vi "01_ui_main_loop.vi"() -> ()   [LabVIEW 2025]
uses:
  0417e9bc-26c0-40a3-857c-749a2451377f.vi
  040e489e-a473-4f93-bd06-0afa5652ce70.vi
  c6e3c1e2-0994-45fa-bff3-5cd5cb70e039.vi
  0bc7f4c2-ffb1-4822-9f64-357063f019c3.vi
  8b609e5e-a51d-4c52-8c18-d6a58a5b9e80.vi
  43d63275-3364-44ab-a9c8-6f7e055a0a8e.vi
  75836779-3642-44ab-91a1-288c14d5bff7.vi
  f856a27e-8979-4d67-ac65-7e3e0066168f.vi
  f6c46c24-e81c-4bed-970f-882e3bbfa33a.vi
  674b8dbc-10ac-464c-a410-8119d69976f5.vi
  efe7b7fb-95db-4648-be1d-36dd24965d64.vi
  a7921508-b016-4ad4-9c73-64ec30acdca8.vi
  2bf2835e-c011-4d5e-a055-403be64c671f.vi
  <vilib>/Utility/config.llb/Read Key (String).vi
  <vilib>/Utility/config.llb/Read Key (U32).vi
  <vilib>/Utility/config.llb/Read Key (Boolean).vi
  <vilib>/Utility/config.llb/Write Key (String).vi
  <vilib>/Utility/config.llb/Write Key (U32).vi
  <vilib>/Utility/config.llb/Write Key (Boolean).vi
  <vilib>/Utility/config.llb/NI_LVConfig.lvlib
panel:
  in  "color_picker_cursor_2":u32(colorbox)=16756736
  in  "color_picker_cursor_1":u32(colorbox)=11927752
  in  "sva_del_cal_file":bool
  in  "sva_cal_file":string(combo)
  in  "button_tcp_load_cal":bool caption="Connect"
  in  "button_tcp_smith_mode":bool caption="Connect"
  in  "button_tcp_s21_mode":bool caption="Connect"
  in  "button_tcp_s11_mode":bool caption="Connect"
  in  "button_tcp_vna_mode":bool caption="Connect"
  in  "show_plot_window":bool
  in  "button_save_s2p":bool caption="Save *.s2p"
  in  "button_tcp_connect":bool caption="Connect"
  in  "sva_port":u16=5025 caption="Port"
  in  "sva_ip":string="192.168.2.29" caption="IP"
  in  "stop":bool
  in  "button_auto_sweep":bool caption="Auto Sweep"
  in  "sweep_points":dbl caption="Points" min=0.0 step=1.0 format="%#_6f"
  in  "sweep_stop":dbl caption="Stop Frequency" min=0.0 step=1.0 format="%#_6f"
  in  "sweep_start":dbl caption="Start Frequency" min=0.0 step=1.0 format="%#_6f"
  in  "selector_serial_port":refnum<visa-resource-name>="COM1" caption="COM-Port"
  out "led_serial_connected":bool caption="Connected"
  in  "button_serial_connect":bool caption="Connect"
  in  "button_single_sweep":bool caption="Single Sweep"
  out "plot_smith_legend_curs_r":dbl caption="Cursor - R"
  out "plot_smith_legend_phase":dbl caption="Phase"
  out "plot_smith_legend_freq":string caption="Frequency"
  out "plot_smith_legend_jx":dbl caption="jX"
  out "plot_smith_legend_r":dbl caption="R"
  out "plot_smith":picture caption="Smith"
  out "filename":string caption="Recent File"
  in  "button_save_s1p":bool caption="Save *.s1p"
  in  "button_load_csv":bool caption="Load *.s1p 2"
  in  "button_load_sxp":bool caption="Load *.sxp"
  in  "show_smith_window":bool
  out "min_vswr_idx":i32
  in  "set_min_vswr_c2":bool
  in  "set_min_vswr_c1":bool
  out "min_vswr_freq":string caption="@ Frequency"
  out "min_vswr":dbl caption="Min. VSWR"
  out "min_frequency":string caption="Min. Frequency"
  out "points":dbl caption="Points"
  out "max_frequency":string caption="Max. Frequency"
  out "plot_smith_legend_curs_x":dbl caption="Cursor - jX"
  out "cursor_cp_1_prefix":string
  out "cursor_lp_1_prefix":string
  out "cursor_cs_1_prefix":string
  out "cursor_ls_1_prefix":string
  out "cursor_cp_2_prefix":string
  out "cursor_lp_2_prefix":string
  out "cursor_cs_2_prefix":string
  in  "lc_scale_settings":enum32{"autoscale", "fancy_scale", "zero_scale"}(radio)=enum."zero_scale"
  out "cursor_ls_2_prefix":string
  out "cursor_cp_2":dbl format="%#_6f"
  in  "color_picker_cp":u32(colorbox)=14468608
  out "cursor_cp_1":dbl format="%#_6f"
  in  "enable_plot_cp":bool=TRUE caption="S11 - Imaginary"
  out "cursor_lp_2":dbl format="%#_6f"
  in  "color_picker_lp":u32(colorbox)=39219
  out "cursor_lp_1":dbl format="%#_6f"
  in  "enable_plot_lp":bool caption="S11 - Imaginary"
  out "cursor_cs_2":dbl format="%#_6f"
  out "cursor_ls_2":dbl format="%#_6f"
  out "cursor_lc_freq_2":string caption="Frequenz"
  out "cursor_lc_wavel_2":dbl caption="Frequenz"
  out "cursor_lc_wavel_1":dbl caption="Frequenz"
  in  "color_picker_cs":u32(colorbox)=14423100
  in  "color_picker_ls":u32(colorbox)=26316
  out "cursor_lc_freq_1":string caption="Frequenz"
  out "cursor_cs_1":dbl format="%#_6f"
  out "cursor_ls_1":dbl format="%#_6f"
  in  "enable_plot_cs":bool caption="S11 - Imaginary"
  in  "enable_plot_ls":bool=TRUE caption="S11 - Real"
  out "plot_lc":cluster{"array type (2D Dbl)":dbl[], dbl[]}[](graph) caption="L+C (Serial) / Lp+Cp (Parallel)"
  out "cursor_z_2":dbl format="%#_6f"
  in  "color_picker_z":u32(colorbox)=13314815
  out "cursor_z_1":dbl format="%#_6f"
  in  "enable_plot_z":bool=TRUE caption="S11 - Imaginary"
  out "cursor_jxp_2":dbl format="%#_6f"
  in  "color_picker_jxp":u32(colorbox)=14468608
  out "cursor_jxp_1":dbl format="%#_6f"
  in  "enable_plot_jxp":bool caption="S11 - Imaginary"
  out "cursor_rp_2":dbl format="%#_6f"
  in  "color_picker_rp":u32(colorbox)=39219
  out "cursor_rp_1":dbl format="%#_6f"
  in  "enable_plot_rp":bool caption="S11 - Imaginary"
  out "cursor_jx_2":dbl format="%#_6f"
  out "cursor_r_2":dbl format="%#_6f"
  out "cursor_imag_2":dbl format="%#_6f"
  out "cursor_real_2":dbl format="%#_6f"
  out "cursor_r_jx_freq_2":string caption="Frequenz"
  out "cursor_r_jx_wavel_2":dbl caption="Frequenz"
  out "cursor_r_jx_wavel_1":dbl caption="Frequenz"
  out "cursor_real_imag_freq_2":string caption="Frequenz"
  out "cursor_real_imag_wavel_2":dbl caption="Frequenz"
  out "cursor_real_imag_wavel_1":dbl caption="Frequenz"
  out "cursor_log_phase_wavel_2":dbl caption="Frequenz"
  out "cursor_log_phase_wavel_1":dbl caption="Frequenz"
  in  "cursor_mode":bool=TRUE caption="Cursor Mode"
  out "cursor_vswr_2":dbl format="%#_6f"
  in  "color_picker_vswr":u32(colorbox)=39219
  out "cursor_vswr_1":dbl format="%#_6f"
  in  "enable_plot_vswr":bool=TRUE caption="S11 - VSWR"
  out "cursor_log_phase_freq_2":string caption="Frequenz"
  out "cursor_phase_2":dbl format="%#_6f"
  out "cursor_logmag_2":dbl format="%#_6f"
  in  "color_picker_jx":u32(colorbox)=14423100
  in  "color_picker_r":u32(colorbox)=26316
  out "cursor_r_jx_freq_1":string caption="Frequenz"
  out "cursor_jx_1":dbl format="%#_6f"
  out "cursor_r_1":dbl format="%#_6f"
  in  "enable_plot_jx":bool=TRUE caption="S11 - Imaginary"
  in  "enable_plot_r":bool=TRUE caption="S11 - Real"
  in  "color_picker_imag":u32(colorbox)=14423100
  in  "color_picker_real":u32(colorbox)=26316
  out "cursor_real_imag_freq_1":string caption="Frequenz"
  out "cursor_imag_1":dbl format="%#_6f"
  out "cursor_real_1":dbl format="%#_6f"
  in  "enable_plot_imag":bool=TRUE caption="S11 - Imaginary"
  in  "enable_plot_real":bool=TRUE caption="S11 - Real"
  out "plot_real_imag":cluster{"array type (2D Dbl)":dbl[], dbl[]}[](graph) caption="Real / Imaginary"
  in  "color_picker_phase":u32(colorbox)=14423100
  in  "color_picker_logmag":u32(colorbox)=26316
  out "cursor_log_phase_freq_1":string caption="Frequenz"
  out "cursor_phase_1":dbl format="%#_6f"
  out "cursor_logmag_1":dbl format="%#_6f"
  in  "rx_scale_settings":enum32{"autoscale", "fancy_scale"}(radio)=enum."fancy_scale"
  in  "enable_plot_phase":bool=TRUE caption="S11 - Phase"
  in  "enable_plot_logmag":bool=TRUE caption="S11 - Logmag"
  out "plot_rjx":cluster{"array type (2D Dbl)":dbl[], dbl[]}[](graph) caption="R+jX (Serial) / Rp+jXp (Parallel) / Z"
  out "plot_log_phase_vswr":cluster{"array type (2D Dbl)":dbl[], dbl[]}[](graph) caption="Logmag / Phase / VSWR"
  # "LabVNA - VNA/S-Parameter Software"
  # "by Robin Tönniges (DC7RT)"
  # "Hz"
  # "NanoVNA"
  # "Siglent SVA"
  # "Sweep"
  # "Trace Data"
  # "Load/Save"
  # "Cursor 1"
  # "Cursor 2"
  # "Frequency"
  # "Hz"
  # "Hz"
  # "Wavelength"
  # "m"
  # "m"
  # "Frequency"
  # "Hz"
  # "Hz"
  # "Wavelength"
  # "m"
  # "m"
  # "Hz"
  # "Frequency"
  # "Hz"
  # "Wavelength"
  # "m"
  # "m"
  # "Frequency [MHz]"
  # "Hz"
  # "Frequency"
  # "Hz"
  # "Wavelength"
  # "m"
  # "m"
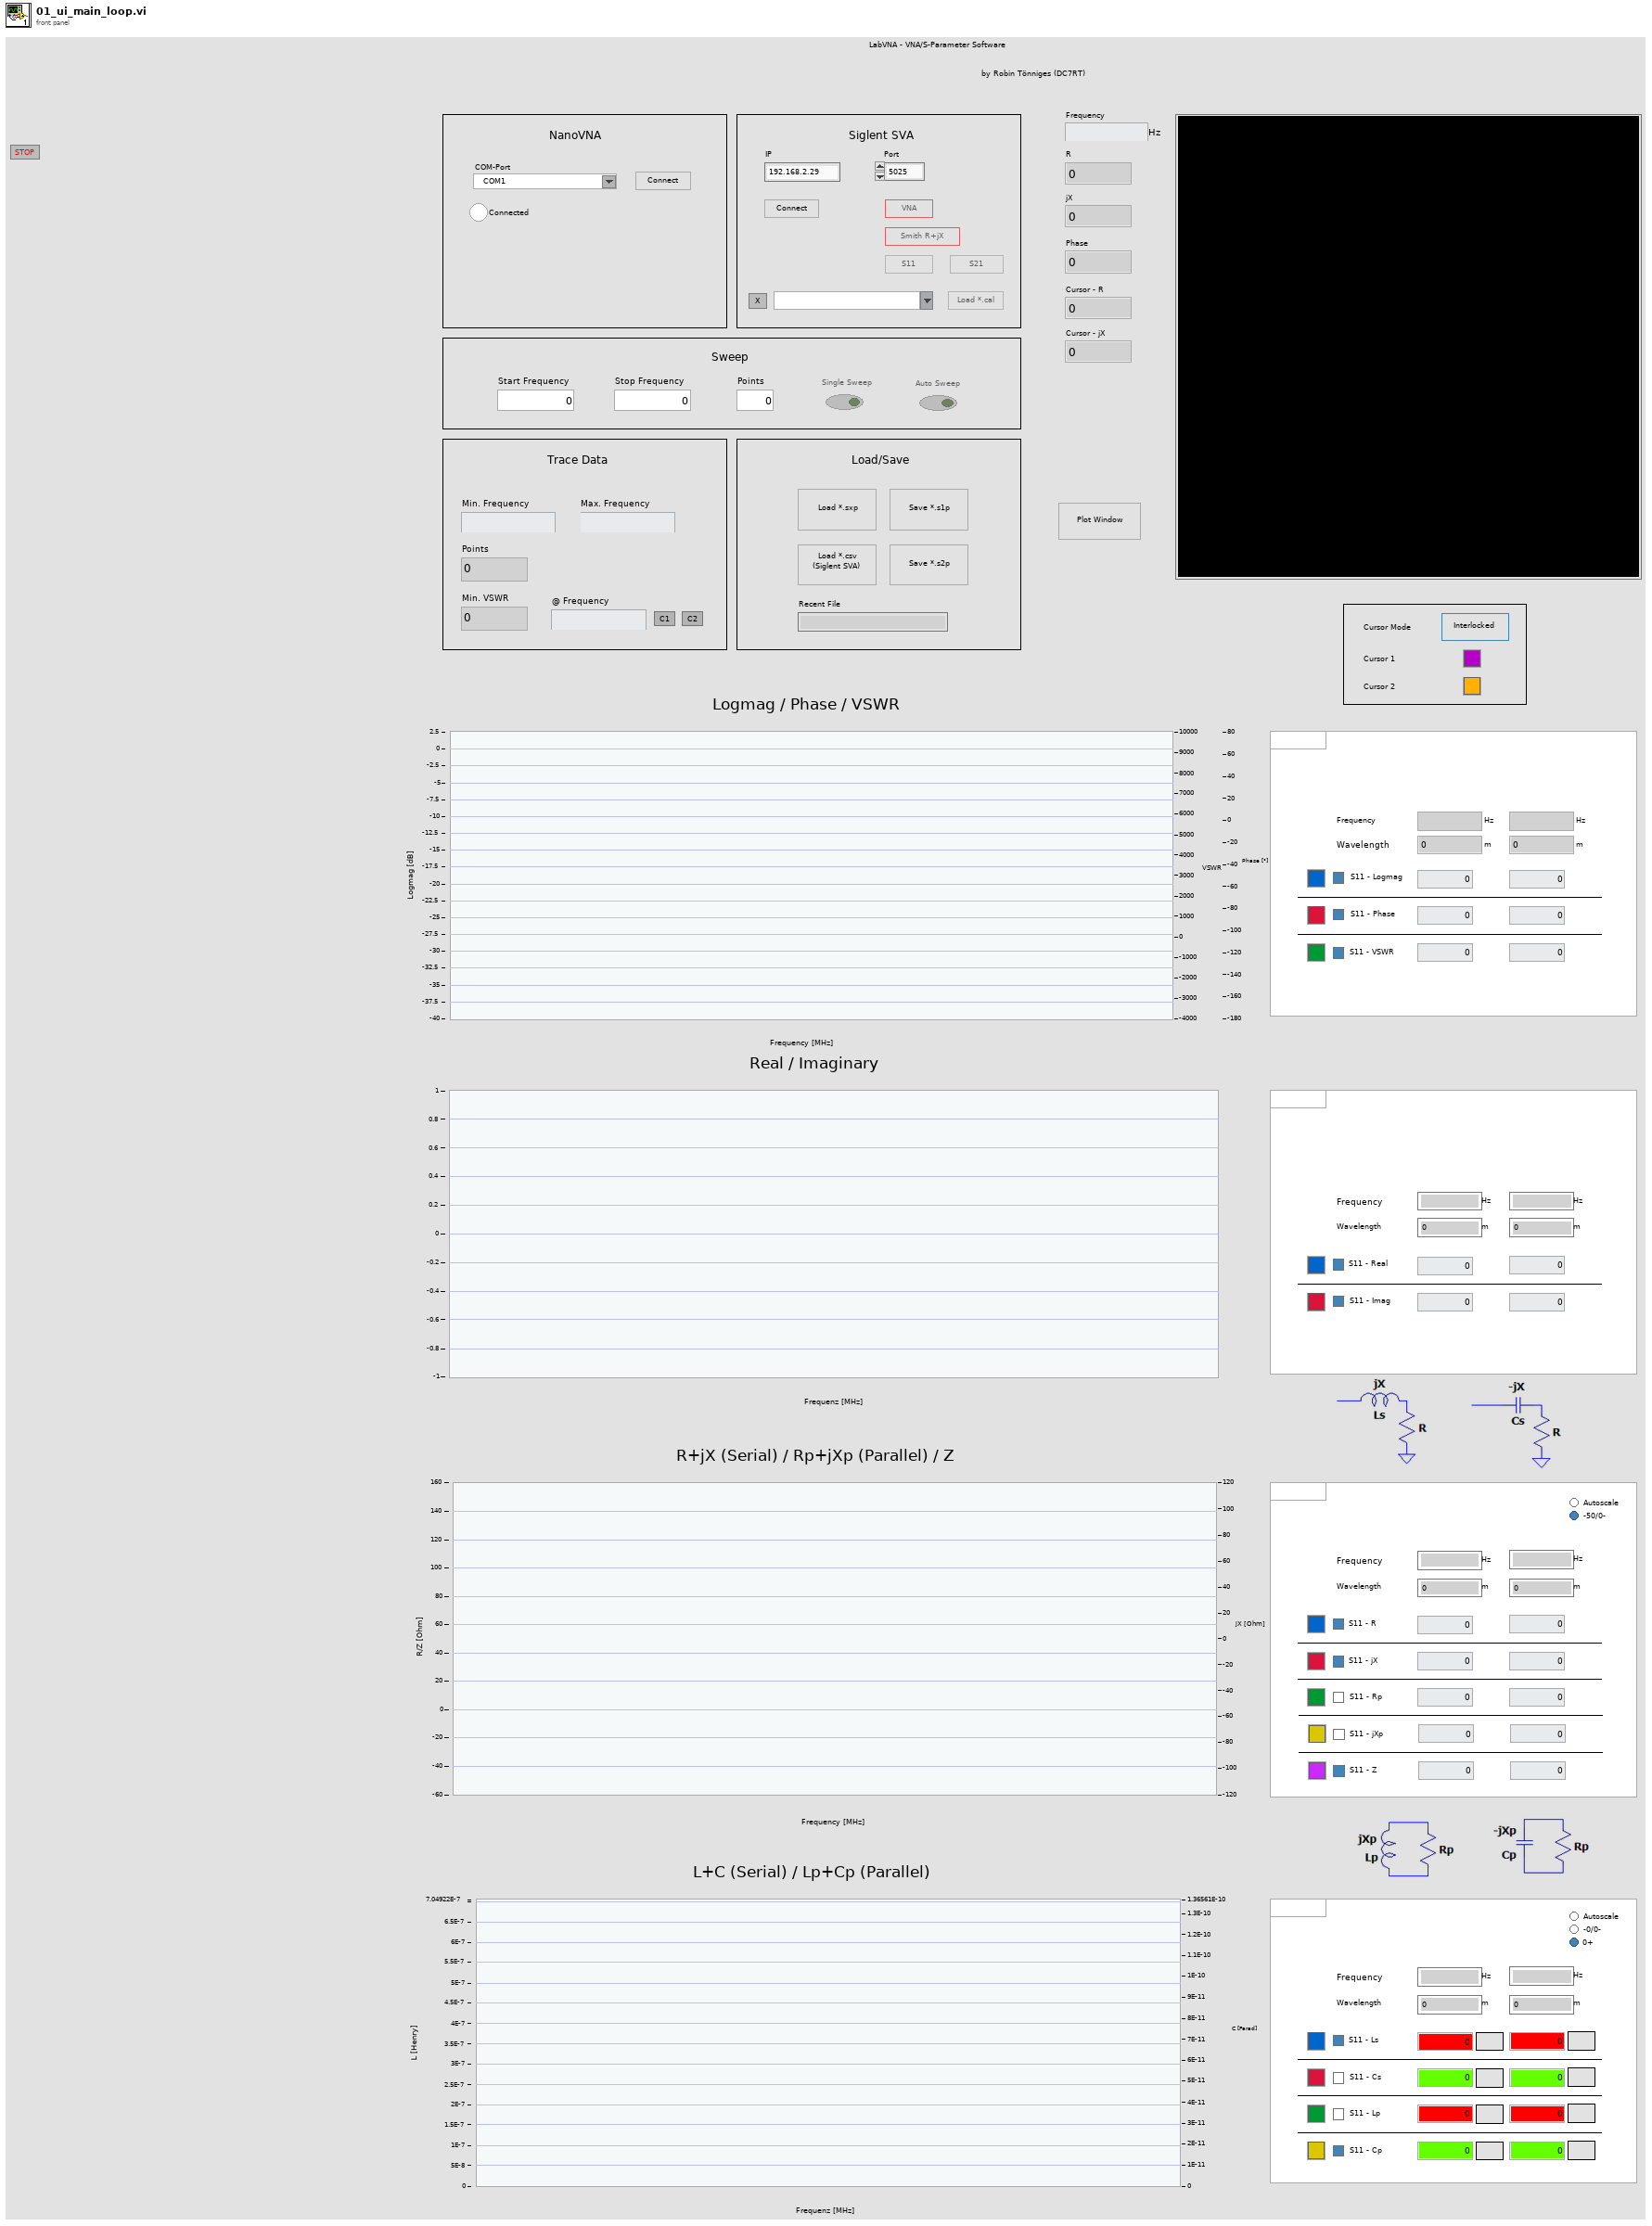
[diagram p1: front panel]
types:
  T1 = cluster{"button_serial_connect":bool, "button_auto_sweep":bool, "button_tcp_connect":bool}
  T2 = cluster{"button_load_sxp":bool, "button_load_csv":bool, "button_save_s1p":bool, "button_save_s2p":bool, "button_single_sweep":bool, "tcp_load_cal":bool, "show_smith_window":bool}
  T3 = enum8{"Enabled", "Disabled", "Disabled and Grayed Out"}
  T4 = enum32{"Invalid", "Standard", "Closed", "Hidden", "Minimized", "Maximized"}
  T5 = cluster{"left":dbl, "top":dbl, "right":dbl, "bottom":dbl}
  T6 = cluster{"x":cluster{"a":dbl, "b":dbl, "log?":bool}, "y":cluster{"a":dbl, "b":dbl, "log?":bool}}
  T7 = typedef "NI_LVConfig.lvlib/Config Data RefNum.ctl" = refnum<k1>
  T8 = cluster{"button_load_sxp":bool, "button_load_csv":bool, "button_save_s1p":bool, "button_save_s2p":bool, "button_single_sweep":bool, "button_tcp_load_cal":bool, "show_smith_window":bool}
  T9 = cluster{"mode":string, "s11_s21":string, "graph":string, "freq_range":cluster{"start_freq":string, "stop_freq":string}, "points":string}
  T10 = typedef "LVCursorListTypeDef.ctl" = cluster{"Name":string, "Color":u32, "Style":u8, "Point Style":u8, "Name Visible":bool, "Allow Drag":bool, "Cursor Mode":u32, "Plot":i32, "Index":i32, "Position":cluster{"X":dbl, "Y":dbl}, "X Scale":u32, "Y Scale":u32, "Watch Plots":i32[], "Watch All Plots":bool, "Plot Area":i32, "Label Offset":cluster{"X":dbl, "Y":dbl}}[]
  T11 = typedef "LVPoint32TypeDef.ctl" = cluster{"Horizontal":i32, "Vertical":i32}
  T12 = cluster{"frequency":dbl, "r":dbl, "jx":dbl, "phase":dbl}
  T13 = cluster{"cursor_data":dbl[], "frequency":string, "wavelength_m":dbl}
  T14 = cluster{"freq_array":dbl[], "data_array":dbl[]}[]
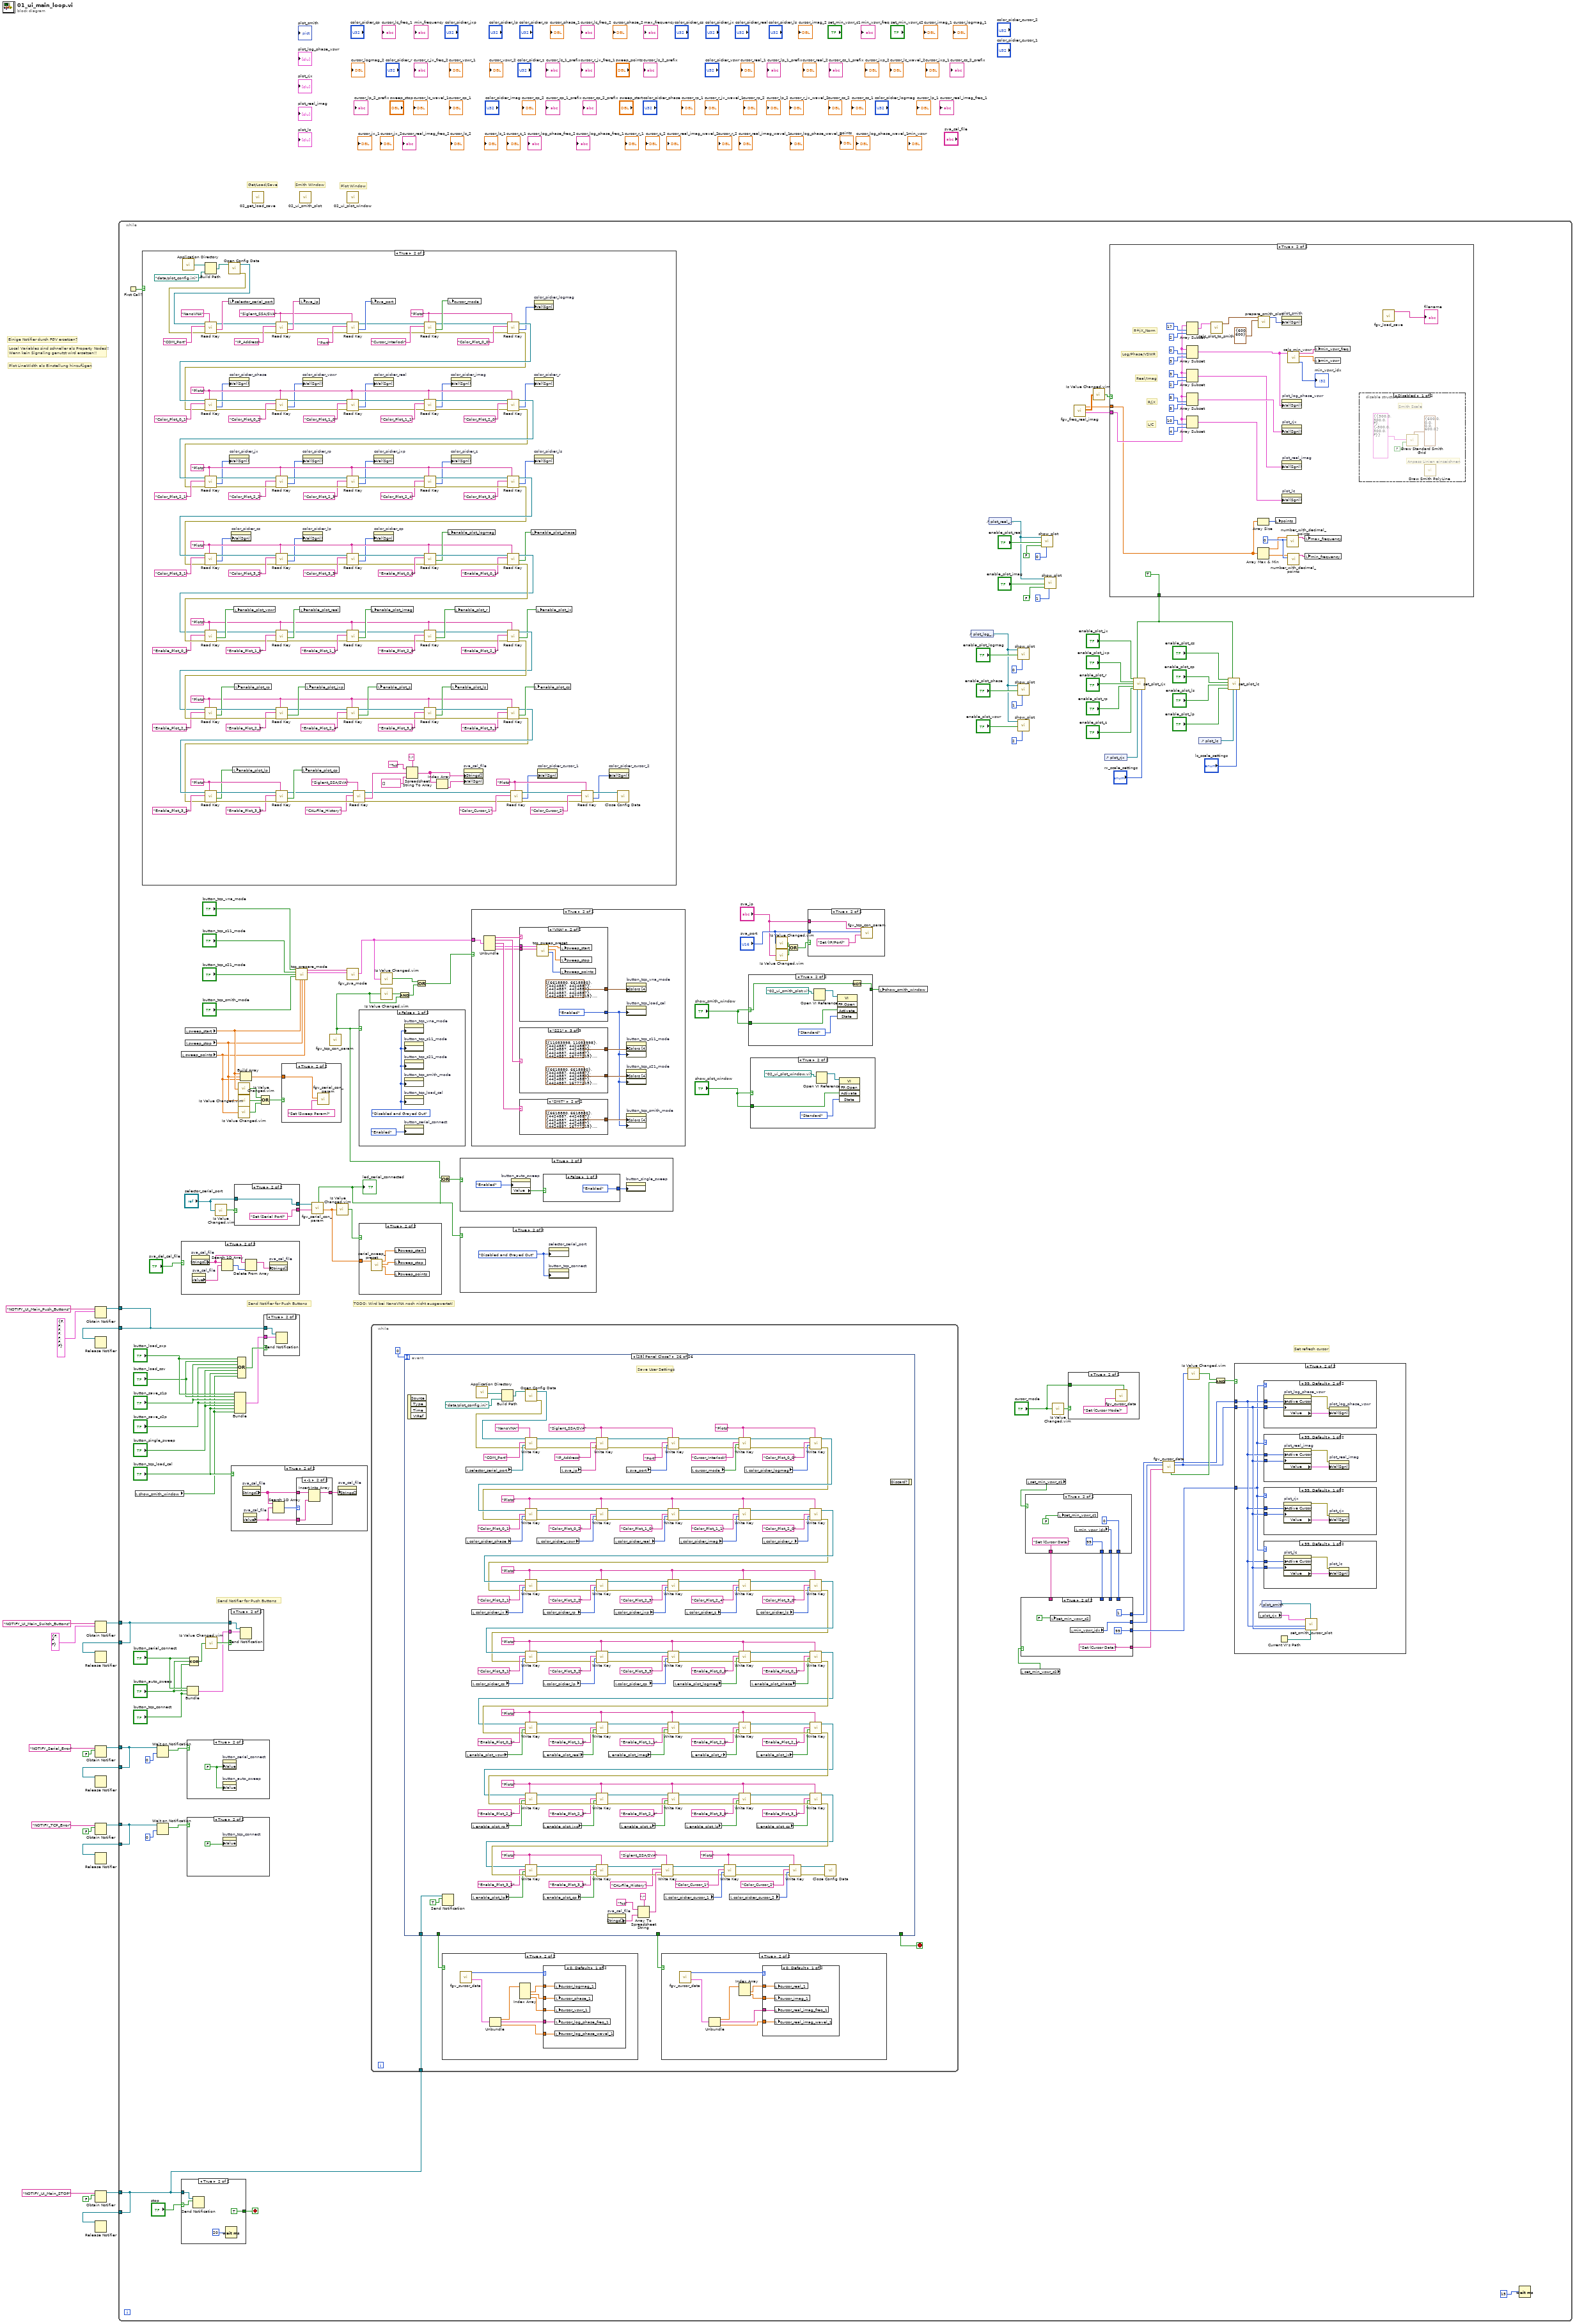
[diagram p0: block diagram]
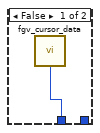
[diagram p9: hidden frame]
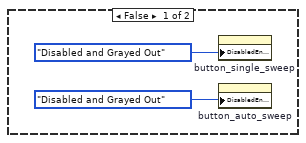
[diagram p11: hidden frame]
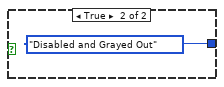
[diagram p12: hidden frame]
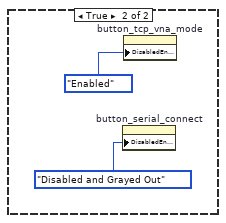
[diagram p16: hidden frame]
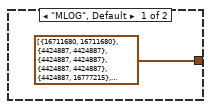
[diagram p18: hidden frame]
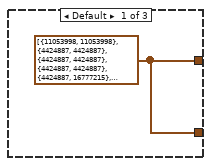
[diagram p19: hidden frame]
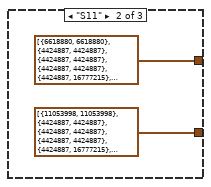
[diagram p20: hidden frame]
diagram:
  # "Plot LineWidth als Einstellung hinzufügen"
  # "Local Variables sind schneller als Property Nodes!!\nWenn kein Signaling genutzt wird ersetzen!!"
  # "Einige Notifier durch FGV ersetzen?"
  # "Plot Window"
  # "Get/Load/Save"
  # "Smith WIndow"
  n1 = Obtain Notifier(name (unnamed)="NOTIFY_UI_Main_Push_Buttons", notification data type=T2 {"button_load_sxp"=FALSE, "button_load_csv"=FALSE, "button_save_s1p"=FALSE, "button_save_s2p"=FALSE, "button_single_sweep"=FALSE, "tcp_load_cal"=FALSE, "show_smith_window"=FALSE} ("output cluster")) -> (notifier out=w19:refnum<notifier>)  [unwired: 2 in, 2 out]
  n2 = Obtain Notifier(name (unnamed)="NOTIFY_UI_Main_Switch_Buttons", notification data type=T1 {"button_serial_connect"=FALSE, "button_auto_sweep"=FALSE, "button_tcp_connect"=FALSE} ("output cluster")) -> (notifier out=w8:refnum<notifier>)  [unwired: 2 in, 2 out]
  n3 = Obtain Notifier(name (unnamed)="NOTIFY_Serial_Error", notification data type=FALSE) -> (notifier out=w11:refnum<notifier>)  [unwired: 2 in, 2 out]
  n4 = Obtain Notifier(name (unnamed)="NOTIFY_TCP_Error", notification data type=FALSE) -> (notifier out=w3:refnum<notifier>)  [unwired: 2 in, 2 out]
  n5 = Obtain Notifier(name (unnamed)="NOTIFY_UI_Main_STOP", notification data type=FALSE) -> (notifier out=w16:refnum<notifier>)  [unwired: 2 in, 2 out]
  n6 = while {
    tunnel: w19 -> [w103]
    tunnel: [w103] -> w18
    tunnel: w16 -> [w80]
    tunnel: [w80] -> w17
    tunnel: w11 -> [w95]
    tunnel: [w95] -> w10
    tunnel: w8 -> [w92]
    tunnel: [w92] -> w9
    tunnel: w3 -> [w63]
    tunnel: [w63] -> w4
    stop <- w96 stop-if-true
    # "Set refresh cursor"
    # "TODO: Wird bei NanoVNA noch nicht ausgewertet!"
    # "Send Notifier for Push Buttons"
    # "Send Notifier for Push Buttons"
    n7 = First Call?() -> (First Call?: T/F=w70:bool)
    n8 = local read "show_smith_window"() -> (w21:bool)
    n9 = case shown="True" w70 {
      frame False {
      }
      frame True {
        w247 = "Plots" ("section")
        w277 = "Plots" ("section")
        w268 = "Plots" ("section")
        w298 = "Plots" ("section")
        w267 = "Plots" ("section")
        w351 = "Plots" ("section")
        w352 = "Plots" ("section")
        w365 = "Plots" ("section")
        w366 = "Siglent_SSA/SVA" ("section")
        n10 = call <vilib>:"Application Directory.vi"() -> ("Application Directory"=w262:path)
        n11 = Build Path(base path=w262, name or relative path=path "data/plot_config.ini") -> (appended path=w266:path)
        n12 = call <vilib>:"Open Config Data.vi"("configuration file path"=w266) -> ("error out"=w264:errorcluster, "refnum"=w263:T7)  [unwired: 8 in, 1 out]
        n13 = call-poly <vilib>:"Read Key.vi"("section"="NanoVNA", "error in (no error)"=w264, "key"="COM_Port", "refnum"=w263) -> ("error out"=w382:errorcluster, "value"=w385:string, "refnum out"=w383:T7)  [unwired: 4 in, 1 out]
        n14 = local write "selector_serial_port"(w385) -> ()
        n15 = call-poly <vilib>:"Read Key.vi"("section"=w366, "error in (no error)"=w382, "key"="IP_Address", "refnum"=w383) -> ("error out"=w378:errorcluster, "value"=w381:string, "refnum out"=w379:T7)  [unwired: 4 in, 1 out]
        n16 = local write "sva_ip"(w381) -> ()
        n17 = call-poly <vilib>:"Read Key.vi"("section"=w366, "error in (no error)"=w378, "key"="Port", "refnum"=w379) -> ("error out"=w374:errorcluster, "value"=w377:u32, "refnum out"=w375:T7)  [unwired: 4 in, 1 out]
        n18 = local write "sva_port"(w377) -> ()
        n19 = call-poly <vilib>:"Read Key.vi"("section"=w365, "error in (no error)"=w374, "key"="Cursor_Interlock", "refnum"=w375) -> ("error out"=w370:errorcluster, "value"=w373:bool, "refnum out"=w371:T7)  [unwired: 4 in, 1 out]
        n20 = local write "cursor_mode"(w373) -> ()
        n21 = call-poly <vilib>:"Read Key.vi"("section"=w365, "error in (no error)"=w370, "key"="Color_Plot_0_0", "refnum"=w371) -> ("error out"=w367:errorcluster, "value"=w242:u32, "refnum out"=w368:T7)  [unwired: 4 in, 1 out]
        n22 = call-poly <vilib>:"Read Key.vi"("section"=w352, "error in (no error)"=w367, "key"="Color_Plot_0_1", "refnum"=w368) -> ("error out"=w362:errorcluster, "value"=w241:u32, "refnum out"=w363:T7)  [unwired: 4 in, 1 out]
        n23 = property on="color_picker_phase" class="ColBox"("Val(Sgnl)"=w241) -> ()  [unwired: 2 in, 2 out]
        n24 = call-poly <vilib>:"Read Key.vi"("section"=w352, "error in (no error)"=w362, "key"="Color_Plot_0_2", "refnum"=w363) -> ("error out"=w359:errorcluster, "value"=w240:u32, "refnum out"=w360:T7)  [unwired: 4 in, 1 out]
        n25 = property on="color_picker_vswr" class="ColBox"("Val(Sgnl)"=w240) -> ()  [unwired: 2 in, 2 out]
        n26 = call-poly <vilib>:"Read Key.vi"("section"=w352, "error in (no error)"=w359, "key"="Color_Plot_1_0", "refnum"=w360) -> ("error out"=w356:errorcluster, "value"=w239:u32, "refnum out"=w357:T7)  [unwired: 4 in, 1 out]
        n27 = property on="color_picker_real" class="ColBox"("Val(Sgnl)"=w239) -> ()  [unwired: 2 in, 2 out]
        n28 = call-poly <vilib>:"Read Key.vi"("section"=w352, "error in (no error)"=w356, "key"="Color_Plot_1_1", "refnum"=w357) -> ("error out"=w353:errorcluster, "value"=w238:u32, "refnum out"=w354:T7)  [unwired: 4 in, 1 out]
        n29 = property on="color_picker_imag" class="ColBox"("Val(Sgnl)"=w238) -> ()  [unwired: 2 in, 2 out]
        n30 = call-poly <vilib>:"Read Key.vi"("section"=w352, "error in (no error)"=w353, "key"="Color_Plot_2_0", "refnum"=w354) -> ("error out"=w336:errorcluster, "value"=w237:u32, "refnum out"=w337:T7)  [unwired: 4 in, 1 out]
        n31 = call-poly <vilib>:"Read Key.vi"("section"=w351, "error in (no error)"=w336, "key"="Color_Plot_2_1", "refnum"=w337) -> ("error out"=w341:errorcluster, "value"=w236:u32, "refnum out"=w340:T7)  [unwired: 4 in, 1 out]
        n32 = property on="color_picker_jx" class="ColBox"("Val(Sgnl)"=w236) -> ()  [unwired: 2 in, 2 out]
        n33 = call-poly <vilib>:"Read Key.vi"("section"=w351, "error in (no error)"=w341, "key"="Color_Plot_2_2", "refnum"=w340) -> ("error out"=w344:errorcluster, "value"=w235:u32, "refnum out"=w343:T7)  [unwired: 4 in, 1 out]
        n34 = property on="color_picker_rp" class="ColBox"("Val(Sgnl)"=w235) -> ()  [unwired: 2 in, 2 out]
        n35 = call-poly <vilib>:"Read Key.vi"("section"=w351, "error in (no error)"=w344, "key"="Color_Plot_2_3", "refnum"=w343) -> ("error out"=w347:errorcluster, "value"=w234:u32, "refnum out"=w346:T7)  [unwired: 4 in, 1 out]
        n36 = property on="color_picker_jxp" class="ColBox"("Val(Sgnl)"=w234) -> ()  [unwired: 2 in, 2 out]
        n37 = call-poly <vilib>:"Read Key.vi"("section"=w351, "error in (no error)"=w347, "key"="Color_Plot_2_4", "refnum"=w346) -> ("error out"=w350:errorcluster, "value"=w233:u32, "refnum out"=w349:T7)  [unwired: 4 in, 1 out]
        n38 = property on="color_picker_z" class="ColBox"("Val(Sgnl)"=w233) -> ()  [unwired: 2 in, 2 out]
        n39 = call-poly <vilib>:"Read Key.vi"("section"=w351, "error in (no error)"=w350, "key"="Color_Plot_3_0", "refnum"=w349) -> ("error out"=w327:errorcluster, "value"=w232:u32, "refnum out"=w328:T7)  [unwired: 4 in, 1 out]
        n40 = call-poly <vilib>:"Read Key.vi"("section"=w267, "error in (no error)"=w327, "key"="Color_Plot_3_1", "refnum"=w328) -> ("error out"=w332:errorcluster, "value"=w231:u32, "refnum out"=w333:T7)  [unwired: 4 in, 1 out]
        n41 = property on="color_picker_cs" class="ColBox"("Val(Sgnl)"=w231) -> ()  [unwired: 2 in, 2 out]
        n42 = call-poly <vilib>:"Read Key.vi"("section"=w267, "error in (no error)"=w332, "key"="Color_Plot_3_2", "refnum"=w333) -> ("error out"=w329:errorcluster, "value"=w230:u32, "refnum out"=w330:T7)  [unwired: 4 in, 1 out]
        n43 = property on="color_picker_lp" class="ColBox"("Val(Sgnl)"=w230) -> ()  [unwired: 2 in, 2 out]
        n44 = call-poly <vilib>:"Read Key.vi"("section"=w267, "error in (no error)"=w329, "key"="Color_Plot_3_3", "refnum"=w330) -> ("error out"=w291:errorcluster, "value"=w229:u32, "refnum out"=w290:T7)  [unwired: 4 in, 1 out]
        n45 = property on="color_picker_cp" class="ColBox"("Val(Sgnl)"=w229) -> ()  [unwired: 2 in, 2 out]
        n46 = call-poly <vilib>:"Read Key.vi"("section"=w267, "error in (no error)"=w291, "key"="Enable_Plot_0_0", "refnum"=w290) -> ("error out"=w296:errorcluster, "value"=w293:bool, "refnum out"=w295:T7)  [unwired: 4 in, 1 out]
        n47 = local write "enable_plot_logmag"(w293) -> ()
        n48 = call-poly <vilib>:"Read Key.vi"("section"=w267, "error in (no error)"=w296, "key"="Enable_Plot_0_1", "refnum"=w295) -> ("error out"=w318:errorcluster, "value"=w297:bool, "refnum out"=w317:T7)  [unwired: 4 in, 1 out]
        n49 = call-poly <vilib>:"Read Key.vi"("section"=w298, "error in (no error)"=w318, "key"="Enable_Plot_0_2", "refnum"=w317) -> ("error out"=w311:errorcluster, "value"=w315:bool, "refnum out"=w312:T7)  [unwired: 4 in, 1 out]
        n50 = local write "enable_plot_vswr"(w315) -> ()
        n51 = call-poly <vilib>:"Read Key.vi"("section"=w298, "error in (no error)"=w311, "key"="Enable_Plot_1_0", "refnum"=w312) -> ("error out"=w307:errorcluster, "value"=w314:bool, "refnum out"=w308:T7)  [unwired: 4 in, 1 out]
        n52 = local write "enable_plot_real"(w314) -> ()
        n53 = call-poly <vilib>:"Read Key.vi"("section"=w298, "error in (no error)"=w307, "key"="Enable_Plot_1_1", "refnum"=w308) -> ("error out"=w303:errorcluster, "value"=w309:bool, "refnum out"=w305:T7)  [unwired: 4 in, 1 out]
        n54 = local write "enable_plot_imag"(w309) -> ()
        n55 = call-poly <vilib>:"Read Key.vi"("section"=w298, "error in (no error)"=w303, "key"="Enable_Plot_2_0", "refnum"=w305) -> ("error out"=w300:errorcluster, "value"=w304:bool, "refnum out"=w301:T7)  [unwired: 4 in, 1 out]
        n56 = local write "enable_plot_r"(w304) -> ()
        n57 = call-poly <vilib>:"Read Key.vi"("section"=w298, "error in (no error)"=w300, "key"="Enable_Plot_2_1", "refnum"=w301) -> ("error out"=w326:errorcluster, "value"=w299:bool, "refnum out"=w325:T7)  [unwired: 4 in, 1 out]
        n58 = call-poly <vilib>:"Read Key.vi"("section"=w268, "error in (no error)"=w326, "key"="Enable_Plot_2_2", "refnum"=w325) -> ("error out"=w324:errorcluster, "value"=w320:bool, "refnum out"=w323:T7)  [unwired: 4 in, 1 out]
        n59 = local write "enable_plot_rp"(w320) -> ()
        n60 = call-poly <vilib>:"Read Key.vi"("section"=w268, "error in (no error)"=w324, "key"="Enable_Plot_2_3", "refnum"=w323) -> ("error out"=w279:errorcluster, "value"=w321:bool, "refnum out"=w278:T7)  [unwired: 4 in, 1 out]
        n61 = local write "enable_plot_jxp"(w321) -> ()
        n62 = call-poly <vilib>:"Read Key.vi"("section"=w268, "error in (no error)"=w279, "key"="Enable_Plot_2_4", "refnum"=w278) -> ("error out"=w285:errorcluster, "value"=w281:bool, "refnum out"=w283:T7)  [unwired: 4 in, 1 out]
        n63 = local write "enable_plot_z"(w281) -> ()
        n64 = call-poly <vilib>:"Read Key.vi"("section"=w268, "error in (no error)"=w285, "key"="Enable_Plot_3_0", "refnum"=w283) -> ("error out"=w288:errorcluster, "value"=w284:bool, "refnum out"=w287:T7)  [unwired: 4 in, 1 out]
        n65 = local write "enable_plot_ls"(w284) -> ()
        n66 = call-poly <vilib>:"Read Key.vi"("section"=w268, "error in (no error)"=w288, "key"="Enable_Plot_3_1", "refnum"=w287) -> ("error out"=w269:errorcluster, "value"=w289:bool, "refnum out"=w270:T7)  [unwired: 4 in, 1 out]
        n67 = call-poly <vilib>:"Read Key.vi"("section"=w277, "error in (no error)"=w269, "key"="Enable_Plot_3_2", "refnum"=w270) -> ("error out"=w276:errorcluster, "value"=w272:bool, "refnum out"=w275:T7)  [unwired: 4 in, 1 out]
        n68 = local write "enable_plot_lp"(w272) -> ()
        n69 = call-poly <vilib>:"Read Key.vi"("section"=w277, "error in (no error)"=w276, "key"="Enable_Plot_3_3", "refnum"=w275) -> ("error out"=w258:errorcluster, "value"=w273:bool, "refnum out"=w259:T7)  [unwired: 4 in, 1 out]
        n70 = local write "enable_plot_cp"(w273) -> ()
        n71 = call-poly <vilib>:"Read Key.vi"("section"="Siglent_SSA/SVA", "error in (no error)"=w258, "key"="CAL-File_History", "refnum"=w259) -> ("error out"=w249:errorcluster, "value"=w261:string, "refnum out"=w250:T7)  [unwired: 4 in, 1 out]
        n72 = Spreadsheet String To Array(delimiter (Tab)=";", format string="%s", spreadsheet string=w261, array type (2D Dbl)=string[] []) -> (array=w253:string[])
        n73 = Index Array(array=w253) -> (element=w252:string)  [unwired: 1 in]
        n74 = property on="sva_cal_file" class="CmbBox"("Strings[]"=w253, "Val(Sgnl)"=w252) -> ()  [unwired: 2 in, 2 out]
        n75 = call-poly <vilib>:"Read Key.vi"("section"=w247, "error in (no error)"=w249, "key"="Color_Cursor_1", "refnum"=w250) -> ("error out"=w243:errorcluster, "value"=w228:u32, "refnum out"=w244:T7)  [unwired: 4 in, 1 out]
        n76 = local write "enable_plot_phase"(w297) -> ()
        n77 = property on="color_picker_logmag" class="ColBox"("Val(Sgnl)"=w242) -> ()  [unwired: 2 in, 2 out]
        n78 = property on="color_picker_r" class="ColBox"("Val(Sgnl)"=w237) -> ()  [unwired: 2 in, 2 out]
        n79 = property on="color_picker_ls" class="ColBox"("Val(Sgnl)"=w232) -> ()  [unwired: 2 in, 2 out]
        n80 = local write "enable_plot_cs"(w289) -> ()
        n81 = local write "enable_plot_jx"(w299) -> ()
        n82 = property on="color_picker_cursor_1" class="ColBox"("Val(Sgnl)"=w228) -> ()  [unwired: 2 in, 2 out]
        n83 = call-poly <vilib>:"Read Key.vi"("section"=w247, "error in (no error)"=w243, "key"="Color_Cursor_2", "refnum"=w244) -> ("error out"=w245:errorcluster, "value"=w227:u32, "refnum out"=w246:T7)  [unwired: 4 in, 1 out]
        n84 = property on="color_picker_cursor_2" class="ColBox"("Val(Sgnl)"=w227) -> ()  [unwired: 2 in, 2 out]
        n85 = call <vilib>:"Close Config Data.vi"("error in (no error)"=w245, "refnum"=w246) -> ()  [unwired: 8 in, 2 out]
      }
    }
    n86 = Wait on Notification(notifier=w95, timeout in ms (-1)=0) -> (notification=w93:bool)  [unwired: 2 in, 3 out]
    n87 = Wait on Notification(notifier=w63, timeout in ms (-1)=0) -> (notification=w65:bool)  [unwired: 2 in, 3 out]
    n88 = case shown="True" "sva_del_cal_file" {
      frame False {
      }
      frame True {
        n89 = property on="sva_cal_file" class="CmbBox"() -> ("Strings[]"=w184:string[])  [unwired: 2 in, 2 out]
        n90 = property on="sva_cal_file" class="CmbBox"() -> ("Value"=w186:string)  [unwired: 2 in, 2 out]
        n91 = Search 1D Array(1D array=w184, element=w186) -> (index of element=w185:i32)  [unwired: 1 in]
        n92 = Delete From Array(array=w184, index=w185) -> (array with subset deleted=w183:string[])  [unwired: 1 in, 1 out]
        n93 = property on="sva_cal_file" class="CmbBox"("Strings[]"=w183) -> ()  [unwired: 2 in, 2 out]
      }
    }
    n94 = case shown="True" "stop" {
      selector: "stop" -> [_ w403]
      tunnel: w80 -> [w399 w404]
      tunnel: [w398 TRUE] -> w96
      frame False {
        n95 = Wait on Notification(notifier=w399, timeout in ms (-1)=0) -> (notification=w398:bool)  [unwired: 2 in, 3 out]
      }
      frame True {
        n96 = Send Notification(notification=w403, notifier=w404) -> ()  [unwired: 1 in, 2 out]
        n97 = Wait (ms)(milliseconds to wait=u32 20) -> ()  [unwired: 1 out]
      }
    }
    n98 = local read "sweep_points"() -> (w40:dbl)
    n99 = local read "sweep_start"() -> (w42:dbl)
    n100 = local read "sweep_stop"() -> (w41:dbl)
    n101 = Bundle("button_serial_connect"="button_serial_connect", "button_auto_sweep"="button_auto_sweep", "button_tcp_connect"="button_tcp_connect") -> (w66:T1)  [unwired: 1 in]
    n102 = case shown="True" w93 {
      frame False {
      }
      frame True {
        w397 = FALSE
        n103 = property on="button_serial_connect" class="Bool (strict)"("Value"=w397) -> ()  [unwired: 2 in, 2 out]
        n104 = property on="button_auto_sweep" class="Bool (strict)"("Value"=w397) -> ()  [unwired: 2 in, 2 out]
      }
    }
    n105 = case shown="True" w65 {
      frame False {
      }
      frame True {
        n106 = property on="button_tcp_connect" class="Bool (strict)"("Value"=FALSE) -> ()  [unwired: 2 in, 2 out]
      }
    }
    n107 = Compound Arithmetic op=XOR("button_serial_connect", "button_auto_sweep", "button_tcp_connect") -> (w87:bool)
    n108 = call "Is Value Changed.vim"("value"=w87) -> ("changed or first call?"=w88:bool)
    n109 = call "Is Value Changed.vim"("value"="selector_serial_port") -> ("changed or first call?"=w132:bool)
    n110 = case shown="True" w88 {
      tunnel: w92 -> [_ w396]
      tunnel: w66 -> [_ w395]
      frame False {
      }
      frame True {
        n111 = Send Notification(notification=w395, notifier=w396) -> ()  [unwired: 1 in, 2 out]
      }
    }
    n112 = case shown="True" "button_tcp_load_cal" {
      frame False {
      }
      frame True {
        n113 = property on="sva_cal_file" class="CmbBox"() -> ("Strings[]"=w189:string[])  [unwired: 2 in, 2 out]
        n114 = property on="sva_cal_file" class="CmbBox"() -> ("Value"=w188:string)  [unwired: 2 in, 2 out]
        n115 = Search 1D Array(1D array=w189, element=w188) -> (index of element=w190:i32)  [unwired: 1 in]
        n116 = case shown="-1" w190 {
          tunnel: w189 -> [w191 w194]
          tunnel: w188 -> [_ w193]
          tunnel: [w191 w192] -> w187
          frame 0, Default {
          }
          frame -1 {
            n117 = Insert Into Array(array=w194, new element=w193) -> (w192:string[])  [unwired: 1 in]
          }
        }
        n118 = property on="sva_cal_file" class="CmbBox"("Strings[]"=w187) -> ()  [unwired: 2 in, 2 out]
      }
    }
    n119 = case shown="True" w132 {
      tunnel: "selector_serial_port" -> [_ w414]
      tunnel: ["Get" ("mode") "Set (Serial Port)" ("mode")] -> w71
      tunnel: [_ w414] -> w72
      frame False {
      }
      frame True {
      }
    }
    n120 = Bundle("button_load_sxp"="button_load_sxp", "button_load_csv"="button_load_csv", "button_save_s1p"="button_save_s1p", "button_save_s2p"="button_save_s2p", "button_single_sweep"="button_single_sweep", "button_tcp_load_cal"="button_tcp_load_cal", "show_smith_window"=w21) -> (w75:T8)  [unwired: 1 in]
    n121 = Compound Arithmetic op=OR("button_load_sxp", "button_load_csv", "button_save_s1p", "button_save_s2p", "button_single_sweep", "button_tcp_load_cal", w21) -> (w98:bool)
    n122 = call "Is Value Changed.vim"("value"=w42) -> ("changed or first call?"=w45:bool)
    n123 = call "Is Value Changed.vim"("value"=w41) -> ("changed or first call?"=w46:bool)
    n124 = call "Is Value Changed.vim"("value"=w40) -> ("changed or first call?"=w44:bool)
    n125 = Build Array(w42, w41, w40) -> (w39:dbl[])
    n126 = Compound Arithmetic op=OR(w45, w46, w44) -> (w43:bool)
    n127 = case shown="True" w98 {
      tunnel: w103 -> [_ w406]
      tunnel: w75 -> [_ w405]
      frame False {
      }
      frame True {
        n128 = Send Notification(notification=w405, notifier=w406) -> ()  [unwired: 1 in, 2 out]
      }
    }
    n129 = case shown="True" w43 {
      tunnel: w39 -> [_ w174]
      frame False {
      }
      frame True {
        n130 = call "fgv_serial_con_param.vi"("mode"="Set (Sweep Param)", "sweep_param_set"=w174) -> ()  [unwired: 5 in, 5 out]
      }
    }
    n131 = call "tcp_prepare_mode.vi"("button_tcp_vna_mode"="button_tcp_vna_mode", "button_tcp_s11_mode"="button_tcp_s11_mode", "button_tcp_s21_mode"="button_tcp_s21_mode", "button_tcp_smith_mode"="button_tcp_smith_mode", "sweep_start"=w42, "sweep_stop"=w41, "sweep_points"=w40) -> ("mode"=w55:string, "data_out"=w54:T9)  [unwired: 7 in]
    n132 = call "fgv_serial_con_param.vi"("mode"=w71, "serial_port_set"=w72) -> ("sweep_param_get"=w73:dbl[], "serial_conn_get"=w48:bool)  [unwired: 5 in, 3 out]
    "led_serial_connected" <- w48
    n133 = call "fgv_tcp_con_param.vi"() -> ("tcp_connected_get"=w47:bool)  [unwired: 8 in, 3 out]
    n134 = call "Is Value Changed.vim"("value"=w73) -> ("changed or first call?"=w130:bool)
    n135 = call "fgv_sva_mode.vi"("data_in"=w54, "mode"=w55) -> ("data_out"=w62:T9)  [unwired: 7 in, 2 out]
    n136 = case shown="False" w47 {
      frame False {
        w196 = T3."Disabled and Grayed Out" ("DisabledEnum")
        n137 = property on="button_tcp_vna_mode" class="Bool"("DisabledEnum"=w196) -> ()  [unwired: 2 in, 2 out]
        n138 = property on="button_tcp_s11_mode" class="Bool"("DisabledEnum"=w196) -> ()  [unwired: 2 in, 2 out]
        n139 = property on="button_tcp_s21_mode" class="Bool"("DisabledEnum"=w196) -> ()  [unwired: 2 in, 2 out]
        n140 = property on="button_tcp_smith_mode" class="Bool"("DisabledEnum"=w196) -> ()  [unwired: 2 in, 2 out]
        n141 = property on="button_tcp_load_cal" class="Bool"("DisabledEnum"=w196) -> ()  [unwired: 2 in, 2 out]
        n142 = property on="button_serial_connect" class="Bool (strict)"("DisabledEnum"=T3."Enabled" ("Disabled")) -> ()  [unwired: 2 in, 2 out]
      }
      frame True {
        n143 = property on="button_serial_connect" class="Bool (strict)"("DisabledEnum"=T3."Disabled and Grayed Out" ("Disabled")) -> ()  [unwired: 2 in, 2 out]
        n144 = property on="button_tcp_vna_mode" class="Bool"("DisabledEnum"=T3."Enabled") -> ()  [unwired: 2 in, 2 out]
      }
    }
    n145 = case shown="True" w130 {
      tunnel: w73 -> [_ w410]
      frame False {
      }
      frame True {
        n146 = call "serial_sweep_preset.vi"("sweep_data"=w410) -> ("sweep_points"=w409:dbl, "sweep_stop"=w408:dbl, "sweep_start"=w407:dbl)  [unwired: 8 in]
        n147 = local write "sweep_start"(w407) -> ()
        n148 = local write "sweep_stop"(w408) -> ()
        n149 = local write "sweep_points"(w409) -> ()
      }
    }
    n150 = while {
      tunnel: w80 -> [w425]
      stop <- w426 stop-if-true
      n151 = event shown="[25] Panel Close?" {
        selector: _ -> [_ _ _ _ _ _ _ _ _ _ _ _ _ _ _ _ _ _ _ _ _ _ _ _ _ _]
        dyn-events: _ -> [_ _ _ _ _ _ _ _ _ _ _ _ _ _ _ _ _ _ _ _ _ _ _ _ _ _]
        timeout: 0 -> [_ _ _ _ _ _ _ _ _ _ _ _ _ _ _ _ _ _ _ _ _ _ _ _ _ _]
        tunnel: [_ _ _ _ _ _ _ _ _ _ _ _ _ _ _ _ _ _ _ _ _ _ _ _ TRUE _] -> w426
        tunnel: w425 -> [_ _ _ _ _ _ _ _ _ _ _ _ _ _ _ _ _ _ _ _ _ _ _ _ _ w977]
        tunnel: [_ _ TRUE _ _ _ _ _ _ _ _ _ _ _ _ _ _ _ _ _ _ _ _ _ _ _] -> w424
        tunnel: [_ _ _ _ _ _ _ TRUE _ _ _ _ _ _ _ _ _ _ _ _ _ _ _ _ _ _] -> w423
        event "color_picker_cursor_1": Value Change {
          w469 = u32 0 ("Active Plot")
          n152 = event-data() -> ("NewVal"=w462:u32)  [unwired: 1 in, 5 out]
          n153 = Bundle("NewVal"=w462, "NewVal"=w462) -> (w463:cluster{"NewVal":u32, "NewVal":u32})  [unwired: 1 in]
          n154 = property on="plot_real_imag" class="XYGraph (strict)"("Active Cursor"=w469, "Cursor.Cursor Color"=w462) -> ()  [unwired: 2 in, 2 out]
          n155 = property on="plot_rjx" class="XYGraph (strict)"("Active Cursor"=w469, "Cursor.Cursor Color"=w462) -> ()  [unwired: 2 in, 2 out]
          n156 = property on="plot_lc" class="XYGraph (strict)"("Active Cursor"=w469, "Cursor.Cursor Color"=w462) -> ()  [unwired: 2 in, 2 out]
          n157 = property on="plot_log_phase_vswr" class="XYGraph (strict)"("Active Cursor"=w469, "Cursor.Cursor Color"=w462) -> ()  [unwired: 2 in, 2 out]
          n158 = property class="VI"() -> (error out=w467:errorcluster, "Front Panel"=w466:refnum<vi>)  [unwired: 2 in, 1 out]
          n159 = call "fgv_cursor_data.vi"("cursor_color_set"=w463, "mode"="Set (Cursor 0 Color)") -> ()  [unwired: 7 in, 7 out]
          n160 = property class="Pnl"(reference=w466, error in=w467) -> ("Decorations[]"=w465:refnum<vi>[])  [unwired: 2 out]
          n161 = Index Array(array=w465, index=0) -> (element=w468:refnum<vi>)
          n162 = property class="Decor"(reference=w468, "BG Color"=w462, "FG Color"=w462) -> ()  [unwired: 1 in, 2 out]
        }
        event "color_picker_cursor_2": Value Change {
          w478 = u32 1 ("Active Plot")
          n163 = event-data() -> ("NewVal"=w470:u32)  [unwired: 1 in, 5 out]
          n164 = Bundle("NewVal"=w470, "NewVal"=w470) -> (w472:cluster{"NewVal":u32, "NewVal":u32})  [unwired: 1 in]
          n165 = property on="plot_real_imag" class="XYGraph (strict)"("Active Cursor"=w478, "Cursor.Cursor Color"=w470) -> ()  [unwired: 2 in, 2 out]
          n166 = property on="plot_rjx" class="XYGraph (strict)"("Active Cursor"=w478, "Cursor.Cursor Color"=w470) -> ()  [unwired: 2 in, 2 out]
          n167 = property on="plot_lc" class="XYGraph (strict)"("Active Cursor"=w478, "Cursor.Cursor Color"=w470) -> ()  [unwired: 2 in, 2 out]
          n168 = property on="plot_log_phase_vswr" class="XYGraph (strict)"("Active Cursor"=w478, "Cursor.Cursor Color"=w470) -> ()  [unwired: 2 in, 2 out]
          n169 = property class="VI"() -> (error out=w476:errorcluster, "Front Panel"=w475:refnum<vi>)  [unwired: 2 in, 1 out]
          n170 = call "fgv_cursor_data.vi"("cursor_color_set"=w472, "mode"="Set (Cursor 1 Color)") -> ()  [unwired: 7 in, 7 out]
          n171 = property class="Pnl"(reference=w475, error in=w476) -> ("Decorations[]"=w474:refnum<vi>[])  [unwired: 2 out]
          n172 = Index Array(array=w474, index=1) -> (element=w477:refnum<vi>)
          n173 = property class="Decor"(reference=w477, "BG Color"=w470, "FG Color"=w470) -> ()  [unwired: 1 in, 2 out]
        }
        event "plot_log_phase_vswr": Cursor Move {
          # "Print Cursor Values for Logmag/Phase-Plot"
          n174 = event-data() -> ("CursIdx"=w483:i32, "CursRef"=w484:refnum<vi>)  [unwired: 1 in, 7 out]
          n175 = property on="Property Node" class="Curs"(reference=w484) -> ("Cursor Index"=w482:i32)  [unwired: 1 in, 2 out]
          n176 = local read "plot_log_phase_vswr"() -> (w480:cluster{"array type (2D Dbl)":dbl[], dbl[]}[])
          n177 = call "fgv_cursor_data.vi"("cursor_idx_set"=w483, "plot_data_set"=w480, "cursor_pos_set"=w482, "mode"="Set (Cursor Data)", "plot_id_set"=0) -> ()  [unwired: 4 in, 7 out]
        }
        event "plot_log_phase_vswr": Value Change {
          # "Print Cursor Values for Logmag/Phase-Plot"
          n178 = event-data() -> ("CtlRef"=w486:refnum<vi>, "NewVal"=w488:cluster{"array type (2D Dbl)":dbl[], dbl[]}[])  [unwired: 1 in, 4 out]
          n179 = property on="Property Node" class="XYGraph (strict)"(reference=w486) -> ("CrsrList"=w487:T10)  [unwired: 1 in, 2 out]
          n180 = Array Size(array=w487) -> (size(s)=w489:i32)
          n181 = for {
            N: w489 -> [_]
            tunnel: w487 -> [w503] mode=indexing
            tunnel: w488 -> [w497]
            i -> [w490]
            n182 = Unbundle By Name(w503) -> ("Index"=w491:i32)
            n183 = call "index_one_axis.vi"("x_index"=w491, "curve_sel"=0 ("x_index"), "graph_data"=w497) -> ("Y"=w494:dbl)  [unwired: 7 in, 1 out]
            n184 = call "index_one_axis.vi"("x_index"=w491, "curve_sel"=1 ("x_index"), "graph_data"=w497) -> ("Y"=w495:dbl)  [unwired: 7 in, 1 out]
            n185 = call "index_one_axis.vi"("x_index"=w491, "curve_sel"=2 ("x_index"), "graph_data"=w497) -> ("Y"=w496:dbl, "X"=w493:dbl)  [unwired: 7 in]
            n186 = call "number_with_decimal_points.vi"("Precision"=i16 0, "Double"=w493) -> ("String"=w502:string)  [unwired: 5 in]
            n187 = call "freq_to_wavelength.vi"("frequency_hz"=w493) -> ("wavelength_m"=w492:dbl)  [unwired: 10 in]
            n188 = case shown="0, Default" w490 {
              tunnel: w502 -> [w508 w513]
              tunnel: w495 -> [w507 w510]
              tunnel: w494 -> [w506 w511]
              tunnel: w496 -> [w505 w512]
              tunnel: w492 -> [w504 w509]
              frame 0, Default {
                n189 = local write "cursor_log_phase_freq_1"(w508) -> ()
                n190 = local write "cursor_log_phase_wavel_1"(w504) -> ()
                n191 = local write "cursor_logmag_1"(w506) -> ()
                n192 = local write "cursor_phase_1"(w507) -> ()
                n193 = local write "cursor_vswr_1"(w505) -> ()
              }
              frame 1 {
                n194 = local write "cursor_log_phase_freq_2"(w513) -> ()
                n195 = local write "cursor_log_phase_wavel_2"(w509) -> ()
                n196 = local write "cursor_phase_2"(w510) -> ()
                n197 = local write "cursor_vswr_2"(w512) -> ()
                n198 = local write "cursor_logmag_2"(w511) -> ()
              }
            }
          }
        }
        event "color_picker_logmag": Value Change {
          # "Change Plot Color Logmag/Phase-Plot [Logmag]"
          n199 = event-data() -> ("NewVal"=w514:u32)  [unwired: 1 in, 5 out]
          n200 = property on="plot_log_phase_vswr" class="XYGraph (strict)"("Active Plot"=u32 0, "Plot.Plot Color"=w514) -> ()  [unwired: 2 in, 2 out]
        }
        event "color_picker_phase": Value Change {
          # "Change Plot Color Logmag/Phase-Plot [Phase]"
          n201 = event-data() -> ("NewVal"=w516:u32)  [unwired: 1 in, 5 out]
          n202 = property on="plot_log_phase_vswr" class="XYGraph (strict)"("Active Plot"=u32 1, "Plot.Plot Color"=w516) -> ()  [unwired: 2 in, 2 out]
        }
        event "color_picker_vswr": Value Change {
          # "Change Plot Color Logmag/Phase-Plot [VSWR]"
          n203 = event-data() -> ("NewVal"=w518:u32)  [unwired: 1 in, 5 out]
          n204 = property on="plot_log_phase_vswr" class="XYGraph (strict)"("Active Plot"=u32 2, "Plot.Plot Color"=w518) -> ()  [unwired: 2 in, 2 out]
        }
        event "plot_real_imag": Cursor Move {
          # "Print Cursor Values for Real/Imag-Plot"
          n205 = event-data() -> ("CursIdx"=w523:i32, "CursRef"=w522:refnum<vi>)  [unwired: 1 in, 7 out]
          n206 = property on="Property Node" class="Curs"(reference=w522) -> ("Cursor Index"=w525:i32)  [unwired: 1 in, 2 out]
          n207 = local read "plot_real_imag"() -> (w521:cluster{"array type (2D Dbl)":dbl[], dbl[]}[])
          n208 = call "fgv_cursor_data.vi"("cursor_idx_set"=w523, "plot_data_set"=w521, "cursor_pos_set"=w525, "mode"="Set (Cursor Data)", "plot_id_set"=1) -> ()  [unwired: 4 in, 7 out]
        }
        event "plot_real_imag": Value Change {
          # "Print Cursor Values for Real/Imag-Plot"
          n209 = event-data() -> ("CtlRef"=w529:refnum<vi>, "NewVal"=w530:cluster{"array type (2D Dbl)":dbl[], dbl[]}[])  [unwired: 1 in, 4 out]
          n210 = property on="Property Node" class="XYGraph (strict)"(reference=w529) -> ("CrsrList"=w527:T10)  [unwired: 1 in, 2 out]
          n211 = Array Size(array=w527) -> (size(s)=w528:i32)
          n212 = for {
            N: w528 -> [_]
            tunnel: w530 -> [w539]
            tunnel: w527 -> [w535] mode=indexing
            i -> [w534]
            n213 = Unbundle By Name(w535) -> ("Index"=w533:i32)
            n214 = call "index_two_axes.vi"("x_index"=w533, "graph_data"=w539) -> ("Y2"=w537:dbl, "Y1"=w538:dbl, "X"=w531:dbl)  [unwired: 7 in]
            n215 = call "number_with_decimal_points.vi"("Precision"=i16 0, "Double"=w531) -> ("String"=w536:string)  [unwired: 5 in]
            n216 = call "freq_to_wavelength.vi"("frequency_hz"=w531) -> ("wavelength_m"=w532:dbl)  [unwired: 10 in]
            n217 = case shown="1" w534 {
              tunnel: w538 -> [w544 w545]
              tunnel: w537 -> [w543 w546]
              tunnel: w536 -> [w542 w547]
              tunnel: w532 -> [w541 w548]
              frame 0, Default {
                n218 = local write "cursor_real_1"(w544) -> ()
                n219 = local write "cursor_imag_1"(w543) -> ()
                n220 = local write "cursor_real_imag_freq_1"(w542) -> ()
                n221 = local write "cursor_real_imag_wavel_1"(w541) -> ()
              }
              frame 1 {
                n222 = local write "cursor_real_imag_freq_2"(w547) -> ()
                n223 = local write "cursor_real_imag_wavel_2"(w548) -> ()
                n224 = local write "cursor_real_2"(w545) -> ()
                n225 = local write "cursor_imag_2"(w546) -> ()
              }
            }
          }
        }
        event "color_picker_real": Value Change {
          n226 = event-data() -> ("NewVal"=w549:u32)  [unwired: 1 in, 5 out]
          n227 = property on="plot_real_imag" class="XYGraph (strict)"("Active Plot"=u32 0, "Plot.Plot Color"=w549) -> ()  [unwired: 2 in, 2 out]
        }
        event "color_picker_imag": Value Change {
          n228 = event-data() -> ("NewVal"=w551:u32)  [unwired: 1 in, 5 out]
          n229 = property on="plot_real_imag" class="XYGraph (strict)"("Active Plot"=u32 1, "Plot.Plot Color"=w551) -> ()  [unwired: 2 in, 2 out]
        }
        event "plot_rjx": Cursor Move {
          # "Print Cursor Values for R/jX-Plot"
          n230 = event-data() -> ("CursIdx"=w556:i32, "CursRef"=w555:refnum<vi>)  [unwired: 1 in, 7 out]
          n231 = property on="Property Node" class="Curs"(reference=w555) -> ("Cursor Index"=w554:i32)  [unwired: 1 in, 2 out]
          n232 = call "fgv_cursor_data.vi"("cursor_idx_set"=w556, "cursor_pos_set"=w554, "mode"="Set (Cursor Data)", "plot_id_set"=2) -> ()  [unwired: 5 in, 7 out]
          n233 = local read "plot_rjx"() -> (w569:cluster{"array type (2D Dbl)":dbl[], dbl[]}[])
          n234 = call "index_one_axis.vi"("x_index"=w554, "curve_sel"=0, "graph_data"=w569) -> ("Y"=w558:dbl)  [unwired: 7 in, 1 out]
          n235 = call "index_one_axis.vi"("x_index"=w554, "curve_sel"=1, "graph_data"=w569) -> ("Y"=w559:dbl)  [unwired: 7 in, 1 out]
          n236 = call "index_one_axis.vi"("x_index"=w554, "curve_sel"=2, "graph_data"=w569) -> ("Y"=w560:dbl)  [unwired: 7 in, 1 out]
          n237 = call "index_one_axis.vi"("x_index"=w554, "curve_sel"=3, "graph_data"=w569) -> ("Y"=w561:dbl)  [unwired: 7 in, 1 out]
          n238 = call "index_one_axis.vi"("x_index"=w554, "curve_sel"=4, "graph_data"=w569) -> ("Y"=w562:dbl, "X"=w563:dbl)  [unwired: 7 in]
          n239 = case shown="1" w556 {
            tunnel: w563 -> [w575 w579]
            tunnel: w562 -> [w574 w580]
            tunnel: w561 -> [w573 w581]
            tunnel: w560 -> [w572 w582]
            tunnel: w559 -> [w571 w583]
            tunnel: w558 -> [w570 w584]
            frame 0, Default {
              n240 = local write "cursor_r_1"(w570) -> ()
              n241 = local write "cursor_jx_1"(w571) -> ()
              n242 = local write "cursor_rp_1"(w572) -> ()
              n243 = local write "cursor_jxp_1"(w573) -> ()
              n244 = local write "cursor_z_1"(w574) -> ()
              n245 = call "number_with_decimal_points.vi"("Precision"=i16 0, "Double"=w575) -> ("String"=w576:string)  [unwired: 5 in]
              n246 = call "freq_to_wavelength.vi"("frequency_hz"=w575) -> ("wavelength_m"=w577:dbl)  [unwired: 10 in]
              n247 = local write "cursor_r_jx_freq_1"(w576) -> ()
              n248 = local write "cursor_r_jx_wavel_1"(w577) -> ()
            }
            frame 1 {
              n249 = local write "cursor_r_2"(w584) -> ()
              n250 = local write "cursor_jx_2"(w583) -> ()
              n251 = local write "cursor_rp_2"(w582) -> ()
              n252 = local write "cursor_jxp_2"(w581) -> ()
              n253 = local write "cursor_z_2"(w580) -> ()
              n254 = call "number_with_decimal_points.vi"("Precision"=i16 0, "Double"=w579) -> ("String"=w586:string)  [unwired: 5 in]
              n255 = call "freq_to_wavelength.vi"("frequency_hz"=w579) -> ("wavelength_m"=w587:dbl)  [unwired: 10 in]
              n256 = local write "cursor_r_jx_freq_2"(w586) -> ()
              n257 = local write "cursor_r_jx_wavel_2"(w587) -> ()
            }
          }
        }
        event "plot_rjx": Value Change {
          # "Print Cursor Values for R/jX-Plot"
          n258 = event-data() -> ("CtlRef"=w590:refnum<vi>, "NewVal"=w588:cluster{"array type (2D Dbl)":dbl[], dbl[]}[])  [unwired: 1 in, 4 out]
          n259 = property on="Property Node" class="XYGraph (strict)"(reference=w590) -> ("CrsrList"=w589:T10)  [unwired: 1 in, 2 out]
          n260 = for {
            tunnel: w589 -> [w602] mode=indexing
            tunnel: w588 -> [w598]
            i -> [w601]
            n261 = Unbundle By Name(w602) -> ("Index"=w597:i32)
            n262 = call "index_five_axes.vi"("x_index"=w597, "graph_data"=w598) -> ("Y4"=w592:dbl, "Y3"=w593:dbl, "Y2"=w594:dbl, "Y1"=w595:dbl, "Y5"=w591:dbl, "X"=w596:dbl)  [unwired: 4 in]
            n263 = call "number_with_decimal_points.vi"("Precision"=i16 0, "Double"=w596) -> ("String"=w600:string)  [unwired: 5 in]
            n264 = call "freq_to_wavelength.vi"("frequency_hz"=w596) -> ("wavelength_m"=w599:dbl)  [unwired: 10 in]
            n265 = case shown="1" w601 {
              tunnel: w600 -> [w610 w616]
              tunnel: w594 -> [w607 w614]
              tunnel: w595 -> [w608 w615]
              tunnel: w599 -> [w609 w617]
              tunnel: w593 -> [w606 w613]
              tunnel: w592 -> [w605 w612]
              tunnel: w591 -> [w604 w611]
              frame 0, Default {
                n266 = local write "cursor_r_jx_freq_1"(w610) -> ()
                n267 = local write "cursor_r_jx_wavel_1"(w609) -> ()
                n268 = local write "cursor_r_1"(w608) -> ()
                n269 = local write "cursor_jx_1"(w607) -> ()
                n270 = local write "cursor_rp_1"(w606) -> ()
                n271 = local write "cursor_jxp_1"(w605) -> ()
                n272 = local write "cursor_z_1"(w604) -> ()
              }
              frame 1 {
                n273 = local write "cursor_r_jx_freq_2"(w616) -> ()
                n274 = local write "cursor_r_jx_wavel_2"(w617) -> ()
                n275 = local write "cursor_r_2"(w615) -> ()
                n276 = local write "cursor_jx_2"(w614) -> ()
                n277 = local write "cursor_rp_2"(w613) -> ()
                n278 = local write "cursor_jxp_2"(w612) -> ()
                n279 = local write "cursor_z_2"(w611) -> ()
              }
            }
          }
        }
        event "color_picker_r": Value Change {
          w619 = u32 0 ("Active Plot")
          # "Change Plot Color R/jX-Plot [R]"
          n280 = event-data() -> ("NewVal"=w618:u32)  [unwired: 1 in, 5 out]
          n281 = property on="plot_rjx" class="XYGraph (strict)"("Active Plot"=w619, "Plot.Plot Color"=w618, "ActYScl"=w619, "YScale.ScaleFit"=w619) -> ()  [unwired: 2 in, 2 out]
        }
        event "color_picker_jx": Value Change {
          w622 = u32 1 ("Active Plot")
          # "Change Plot Color R/jX-Plot [jX]"
          n282 = event-data() -> ("NewVal"=w620:u32)  [unwired: 1 in, 5 out]
          n283 = property on="plot_rjx" class="XYGraph (strict)"("Active Plot"=w622, "Plot.Plot Color"=w620, "ActYScl"=w622, "YScale.ScaleFit"=u8 0 ("Y Scale.Scale Fit")) -> ()  [unwired: 2 in, 2 out]
        }
        event "color_picker_rp": Value Change {
          # "Change Plot Color R/jX-Plot [Rp]"
          n284 = event-data() -> ("NewVal"=w623:u32)  [unwired: 1 in, 5 out]
          n285 = property on="plot_rjx" class="XYGraph (strict)"("Active Plot"=u32 2, "Plot.Plot Color"=w623, "ActYScl"=u32 0 ("Active Plot"), "YScale.ScaleFit"=u8 0 ("Y Scale.Scale Fit")) -> ()  [unwired: 2 in, 2 out]
        }
        event "color_picker_jxp": Value Change {
          # "Change Plot Color R/jX-Plot [jXp]"
          n286 = event-data() -> ("NewVal"=w627:u32)  [unwired: 1 in, 5 out]
          n287 = property on="plot_rjx" class="XYGraph (strict)"("Active Plot"=u32 3, "Plot.Plot Color"=w627, "ActYScl"=u32 1 ("Active Plot"), "YScale.ScaleFit"=u8 0 ("Y Scale.Scale Fit")) -> ()  [unwired: 2 in, 2 out]
        }
        event "color_picker_z": Value Change {
          # "Change Plot Color R/jX-Plot [Z]"
          n288 = event-data() -> ("NewVal"=w631:u32)  [unwired: 1 in, 5 out]
          n289 = property on="plot_rjx" class="XYGraph (strict)"("Active Plot"=u32 4, "Plot.Plot Color"=w631, "ActYScl"=u32 0 ("Active Plot"), "YScale.ScaleFit"=u8 0 ("Y Scale.Scale Fit")) -> ()  [unwired: 2 in, 2 out]
        }
        event "plot_lc": Cursor Move {
          w652 = "F" ("unit")
          w651 = "H" ("unit")
          # "Print Cursor Values for R/jX-Plot"
          n290 = event-data() -> ("CursIdx"=w638:i32, "CursRef"=w637:refnum<vi>)  [unwired: 1 in, 7 out]
          n291 = property on="Property Node" class="Curs"(reference=w637) -> ("Cursor Index"=w636:i32)  [unwired: 1 in, 2 out]
          n292 = local read "plot_lc"() -> (w653:cluster{"array type (2D Dbl)":dbl[], dbl[]}[])
          n293 = call "fgv_cursor_data.vi"("cursor_idx_set"=w638, "cursor_pos_set"=w636, "mode"="Set (Cursor Data)", "plot_id_set"=3) -> ()  [unwired: 5 in, 7 out]
          n294 = call "index_four_axes.vi"("x_index"=w636, "graph_data"=w653) -> ("Y4"=w658:dbl, "Y3"=w657:dbl, "Y2"=w655:dbl, "Y1"=w654:dbl, "X"=w656:dbl)  [unwired: 5 in]
          n295 = call "number_with_decimal_points.vi"("Precision"=i16 0, "Double"=w656) -> ("String"=w649:string)  [unwired: 5 in]
          n296 = call "freq_to_wavelength.vi"("frequency_hz"=w656) -> ("wavelength_m"=w648:dbl)  [unwired: 10 in]
          n297 = call "calc_prefix.vi"("unit"=w651, "Numeric in"=w654) -> ("prefix"=w646:string, "Numeric out"=w647:dbl)  [unwired: 8 in]
          n298 = call "calc_prefix.vi"("unit"=w652, "Numeric in"=w655) -> ("prefix"=w644:string, "Numeric out"=w645:dbl)  [unwired: 8 in]
          n299 = call "calc_prefix.vi"("unit"=w651, "Numeric in"=w657) -> ("prefix"=w642:string, "Numeric out"=w643:dbl)  [unwired: 8 in]
          n300 = call "calc_prefix.vi"("unit"=w652, "Numeric in"=w658) -> ("prefix"=w640:string, "Numeric out"=w641:dbl)  [unwired: 8 in]
          n301 = case shown="0, Default" w638 {
            tunnel: w649 -> [w672 w685]
            tunnel: w648 -> [w671 w686]
            tunnel: w647 -> [w670 w687]
            tunnel: w646 -> [w669 w688]
            tunnel: w645 -> [w667 w689]
            tunnel: w644 -> [w666 w690]
            tunnel: w643 -> [w664 w691]
            tunnel: w642 -> [w662 w693]
            tunnel: w641 -> [w661 w692]
            tunnel: w640 -> [w660 w694]
            frame 0, Default {
              n302 = local write "cursor_lc_freq_1"(w672) -> ()
              n303 = local write "cursor_lc_wavel_1"(w671) -> ()
              n304 = local write "cursor_ls_1"(w670) -> ()
              n305 = local write "cursor_ls_1_prefix"(w669) -> ()
              n306 = local write "cursor_cs_1"(w667) -> ()
              n307 = local write "cursor_cs_1_prefix"(w666) -> ()
              n308 = local write "cursor_lp_1"(w664) -> ()
              n309 = local write "cursor_lp_1_prefix"(w662) -> ()
              n310 = local write "cursor_cp_1"(w661) -> ()
              n311 = local write "cursor_cp_1_prefix"(w660) -> ()
              n312 = Less Than 0?(x=w670) -> (x < 0?=w676:bool)
              n313 = Less Than 0?(x=w667) -> (x < 0?=w675:bool)
              n314 = Less Than 0?(x=w664) -> (x < 0?=w674:bool)
              n315 = Less Than 0?(x=w661) -> (x < 0?=w673:bool)
              n316 = case shown="False" w676 {
                tunnel: [u32 6618880 ("Label.BG Color") u32 16711680 ("Label.BG Color")] -> w668
                frame False {
                }
                frame True {
                }
              }
              n317 = case shown="False" w675 {
                tunnel: [u32 6618880 ("Label.BG Color") u32 16711680 ("Label.BG Color")] -> w665
                frame False {
                }
                frame True {
                }
              }
              n318 = case shown="False" w674 {
                tunnel: [u32 6618880 ("Label.BG Color") u32 16711680 ("Label.BG Color")] -> w663
                frame False {
                }
                frame True {
                }
              }
              n319 = case shown="False" w673 {
                tunnel: [u32 6618880 ("Label.BG Color") u32 16711680 ("Label.BG Color")] -> w659
                frame False {
                }
                frame True {
                }
              }
              n320 = property on="cursor_ls_1" class="DigNum (strict)"("NumText.BGColor"=w668) -> ()  [unwired: 2 in, 2 out]
              n321 = property on="cursor_cs_1" class="DigNum (strict)"("NumText.BGColor"=w665) -> ()  [unwired: 2 in, 2 out]
              n322 = property on="cursor_lp_1" class="DigNum (strict)"("NumText.BGColor"=w663) -> ()  [unwired: 2 in, 2 out]
              n323 = property on="cursor_cp_1" class="DigNum (strict)"("NumText.BGColor"=w659) -> ()  [unwired: 2 in, 2 out]
            }
            frame 1 {
              n324 = local write "cursor_lc_freq_2"(w685) -> ()
              n325 = local write "cursor_lc_wavel_2"(w686) -> ()
              n326 = local write "cursor_ls_2"(w687) -> ()
              n327 = local write "cursor_ls_2_prefix"(w688) -> ()
              n328 = local write "cursor_cs_2"(w689) -> ()
              n329 = local write "cursor_cs_2_prefix"(w690) -> ()
              n330 = local write "cursor_lp_2"(w691) -> ()
              n331 = local write "cursor_lp_2_prefix"(w693) -> ()
              n332 = local write "cursor_cp_2"(w692) -> ()
              n333 = local write "cursor_cp_2_prefix"(w694) -> ()
              n334 = Less Than 0?(x=w687) -> (x < 0?=w702:bool)
              n335 = Less Than 0?(x=w689) -> (x < 0?=w701:bool)
              n336 = Less Than 0?(x=w691) -> (x < 0?=w700:bool)
              n337 = Less Than 0?(x=w692) -> (x < 0?=w699:bool)
              n338 = case shown="False" w702 {
                tunnel: [u32 6618880 ("Label.BG Color") u32 16711680 ("Label.BG Color")] -> w698
                frame False {
                }
                frame True {
                }
              }
              n339 = case shown="False" w701 {
                tunnel: [u32 6618880 ("Label.BG Color") u32 16711680 ("Label.BG Color")] -> w697
                frame False {
                }
                frame True {
                }
              }
              n340 = case shown="False" w700 {
                tunnel: [u32 6618880 ("Label.BG Color") u32 16711680 ("Label.BG Color")] -> w696
                frame False {
                }
                frame True {
                }
              }
              n341 = case shown="False" w699 {
                tunnel: [u32 6618880 ("Label.BG Color") u32 16711680 ("Label.BG Color")] -> w695
                frame False {
                }
                frame True {
                }
              }
              n342 = property on="cursor_ls_2" class="DigNum (strict)"("NumText.BGColor"=w698) -> ()  [unwired: 2 in, 2 out]
              n343 = property on="cursor_cs_2" class="DigNum (strict)"("NumText.BGColor"=w697) -> ()  [unwired: 2 in, 2 out]
              n344 = property on="cursor_lp_2" class="DigNum (strict)"("NumText.BGColor"=w696) -> ()  [unwired: 2 in, 2 out]
              n345 = property on="cursor_cp_2" class="DigNum (strict)"("NumText.BGColor"=w695) -> ()  [unwired: 2 in, 2 out]
            }
          }
        }
        event "plot_lc": Value Change {
          n346 = event-data() -> ("CtlRef"=w712:refnum<vi>, "NewVal"=w711:cluster{"array type (2D Dbl)":dbl[], dbl[]}[])  [unwired: 1 in, 4 out]
          n347 = property on="Property Node" class="XYGraph (strict)"(reference=w712) -> ("CrsrList"=w713:T10)  [unwired: 1 in, 2 out]
          n348 = Array Size(array=w713) -> (size(s)=w714:i32)
          n349 = for {
            N: w714 -> [_]
            tunnel: w713 -> [w735] mode=indexing
            tunnel: w711 -> [w734]
            i -> [w725]
            w726 = "H" ("unit")
            w727 = "F" ("unit")
            n350 = Unbundle By Name(w735) -> ("Index"=w733:i32)
            n351 = call "index_four_axes.vi"("x_index"=w733, "graph_data"=w734) -> ("Y4"=w728:dbl, "Y3"=w729:dbl, "Y2"=w730:dbl, "Y1"=w731:dbl, "X"=w732:dbl)  [unwired: 5 in]
            n352 = call "number_with_decimal_points.vi"("Precision"=i16 0, "Double"=w732) -> ("String"=w715:string)  [unwired: 5 in]
            n353 = call "freq_to_wavelength.vi"("frequency_hz"=w732) -> ("wavelength_m"=w716:dbl)  [unwired: 10 in]
            n354 = call "calc_prefix.vi"("unit"=w726, "Numeric in"=w731) -> ("prefix"=w718:string, "Numeric out"=w717:dbl)  [unwired: 8 in]
            n355 = call "calc_prefix.vi"("unit"=w727, "Numeric in"=w730) -> ("prefix"=w720:string, "Numeric out"=w719:dbl)  [unwired: 8 in]
            n356 = call "calc_prefix.vi"("unit"=w726, "Numeric in"=w729) -> ("prefix"=w722:string, "Numeric out"=w721:dbl)  [unwired: 8 in]
            n357 = call "calc_prefix.vi"("unit"=w727, "Numeric in"=w728) -> ("prefix"=w724:string, "Numeric out"=w723:dbl)  [unwired: 8 in]
            n358 = case shown="1" w725 {
              tunnel: w715 -> [w750 w763]
              tunnel: w716 -> [w749 w764]
              tunnel: w717 -> [w748 w765]
              tunnel: w718 -> [w747 w766]
              tunnel: w719 -> [w745 w767]
              tunnel: w720 -> [w744 w768]
              tunnel: w721 -> [w742 w769]
              tunnel: w722 -> [w740 w771]
              tunnel: w723 -> [w739 w770]
              tunnel: w724 -> [w738 w772]
              frame 0, Default {
                n359 = local write "cursor_lc_freq_1"(w750) -> ()
                n360 = local write "cursor_lc_wavel_1"(w749) -> ()
                n361 = local write "cursor_ls_1"(w748) -> ()
                n362 = local write "cursor_ls_1_prefix"(w747) -> ()
                n363 = local write "cursor_cs_1"(w745) -> ()
                n364 = local write "cursor_cs_1_prefix"(w744) -> ()
                n365 = local write "cursor_lp_1"(w742) -> ()
                n366 = local write "cursor_lp_1_prefix"(w740) -> ()
                n367 = local write "cursor_cp_1"(w739) -> ()
                n368 = local write "cursor_cp_1_prefix"(w738) -> ()
                n369 = Less Than 0?(x=w748) -> (x < 0?=w754:bool)
                n370 = Less Than 0?(x=w745) -> (x < 0?=w753:bool)
                n371 = Less Than 0?(x=w742) -> (x < 0?=w752:bool)
                n372 = Less Than 0?(x=w739) -> (x < 0?=w751:bool)
                n373 = case shown="False" w754 {
                  tunnel: [u32 6618880 ("Label.BG Color") u32 16711680 ("Label.BG Color")] -> w746
                  frame False {
                  }
                  frame True {
                  }
                }
                n374 = case shown="False" w753 {
                  tunnel: [u32 6618880 ("Label.BG Color") u32 16711680 ("Label.BG Color")] -> w743
                  frame False {
                  }
                  frame True {
                  }
                }
                n375 = case shown="False" w752 {
                  tunnel: [u32 6618880 ("Label.BG Color") u32 16711680 ("Label.BG Color")] -> w741
                  frame False {
                  }
                  frame True {
                  }
                }
                n376 = case shown="False" w751 {
                  tunnel: [u32 6618880 ("Label.BG Color") u32 16711680 ("Label.BG Color")] -> w737
                  frame False {
                  }
                  frame True {
                  }
                }
                n377 = property on="cursor_ls_1" class="DigNum (strict)"("NumText.BGColor"=w746) -> ()  [unwired: 2 in, 2 out]
                n378 = property on="cursor_cs_1" class="DigNum (strict)"("NumText.BGColor"=w743) -> ()  [unwired: 2 in, 2 out]
                n379 = property on="cursor_lp_1" class="DigNum (strict)"("NumText.BGColor"=w741) -> ()  [unwired: 2 in, 2 out]
                n380 = property on="cursor_cp_1" class="DigNum (strict)"("NumText.BGColor"=w737) -> ()  [unwired: 2 in, 2 out]
              }
              frame 1 {
                n381 = local write "cursor_lc_freq_2"(w763) -> ()
                n382 = local write "cursor_lc_wavel_2"(w764) -> ()
                n383 = local write "cursor_ls_2"(w765) -> ()
                n384 = local write "cursor_ls_2_prefix"(w766) -> ()
                n385 = local write "cursor_cs_2"(w767) -> ()
                n386 = local write "cursor_cs_2_prefix"(w768) -> ()
                n387 = local write "cursor_lp_2"(w769) -> ()
                n388 = local write "cursor_lp_2_prefix"(w771) -> ()
                n389 = local write "cursor_cp_2"(w770) -> ()
                n390 = local write "cursor_cp_2_prefix"(w772) -> ()
                n391 = Less Than 0?(x=w765) -> (x < 0?=w780:bool)
                n392 = Less Than 0?(x=w767) -> (x < 0?=w779:bool)
                n393 = Less Than 0?(x=w769) -> (x < 0?=w778:bool)
                n394 = Less Than 0?(x=w770) -> (x < 0?=w777:bool)
                n395 = case shown="False" w780 {
                  tunnel: [u32 6618880 ("Label.BG Color") u32 16711680 ("Label.BG Color")] -> w776
                  frame False {
                  }
                  frame True {
                  }
                }
                n396 = case shown="False" w779 {
                  tunnel: [u32 6618880 ("Label.BG Color") u32 16711680 ("Label.BG Color")] -> w775
                  frame False {
                  }
                  frame True {
                  }
                }
                n397 = case shown="False" w778 {
                  tunnel: [u32 6618880 ("Label.BG Color") u32 16711680 ("Label.BG Color")] -> w774
                  frame False {
                  }
                  frame True {
                  }
                }
                n398 = case shown="False" w777 {
                  tunnel: [u32 6618880 ("Label.BG Color") u32 16711680 ("Label.BG Color")] -> w773
                  frame False {
                  }
                  frame True {
                  }
                }
                n399 = property on="cursor_ls_2" class="DigNum (strict)"("NumText.BGColor"=w776) -> ()  [unwired: 2 in, 2 out]
                n400 = property on="cursor_cs_2" class="DigNum (strict)"("NumText.BGColor"=w775) -> ()  [unwired: 2 in, 2 out]
                n401 = property on="cursor_lp_2" class="DigNum (strict)"("NumText.BGColor"=w774) -> ()  [unwired: 2 in, 2 out]
                n402 = property on="cursor_cp_2" class="DigNum (strict)"("NumText.BGColor"=w773) -> ()  [unwired: 2 in, 2 out]
              }
            }
          }
        }
        event "plot_smith": Mouse Move {
          w805 = 300 ("top_center")
          # "Print Mouse-Cursor Values for Smith-Plot"
          n403 = event-data() -> ("Coords"=w806:T11)  [unwired: 1 in, 4 out]
          n404 = local read "plot_log_phase_vswr"() -> (w804:cluster{"array type (2D Dbl)":dbl[], dbl[]}[])
          n405 = local read "plot_real_imag"() -> (w801:cluster{"array type (2D Dbl)":dbl[], dbl[]}[])
          n406 = local read "plot_rjx"() -> (w802:cluster{"array type (2D Dbl)":dbl[], dbl[]}[])
          n407 = property on="plot_smith" class="Pict"() -> ("Top"=w790:i32, "Left"=w789:i32)  [unwired: 2 in, 2 out]
          n408 = Insert Into Array(array=w802, new element=w804) -> (w803:cluster{"array type (2D Dbl)":dbl[], dbl[]}[])  [unwired: 1 in]
          n409 = call "get_smith_hover.vi"("smith_pos_left"=w789, "left_center"=w805, "smith_pos_top"=w790, "top_center"=w805, "Coords"=w806, "cursor_data"=w803, "ref_data"=w801) -> ("cursor_pos"=w799:cluster{"r_norm":dbl, "x_norm":dbl}, "cursor_data"=w800:T12)  [unwired: 3 in]
          n410 = Unbundle(w800) -> ("frequency"=w797:dbl, "r"=→"plot_smith_legend_r":dbl, "jx"=→"plot_smith_legend_jx":dbl, "phase"=→"plot_smith_legend_phase":dbl)
          n411 = Unbundle(w799) -> ("r_norm"=→"plot_smith_legend_curs_r":dbl, "x_norm"=→"plot_smith_legend_curs_x":dbl)
          n412 = call "number_with_decimal_points.vi"("Precision"=i16 0, "Double"=w797) -> ("String"=→"plot_smith_legend_freq":string)  [unwired: 5 in]
        }
        event "plot_smith": Mouse Up {
          # "Show separate Smith Plot"
          n413 = event-data() -> ()  [unwired: 1 in, 8 out]
          n414 = property on="show_smith_window" class="Bool (strict)"("Value"=TRUE ("Boolean")) -> ()  [unwired: 2 in, 2 out]
        }
        event "plot_smith": Value Change {
          n415 = event-data() -> ()  [unwired: 1 in, 6 out]
          n416 = property on="plot_log_phase_vswr" class="XYGraph (strict)"() -> ("CrsrList"=w808:T10)  [unwired: 2 in, 2 out]
          n417 = for {
            tunnel: w808 -> [w812] mode=indexing
            i -> [w811]
            n418 = local read "plot_rjx"() -> (w813:cluster{"array type (2D Dbl)":dbl[], dbl[]}[])
            n419 = control-ref of="plot_smith"() -> (w809:refnum<vi>)
            n420 = Unbundle By Name(w812) -> ("Index"=w810:i32)
            n421 = Current VI's Path() -> (path=w814:path)
            n422 = call "set_smith_cursor_plot.vi"("path"=w814, "smith_plot"=w809, "cursor_pos"=w810, "cursor_index"=w811, "plot_rjx"=w813) -> ()  [unwired: 7 in]
          }
        }
        event "sva_cal_file": Value Change {
          n423 = event-data() -> ("NewVal"=w816:string)  [unwired: 1 in, 5 out]
          n424 = call "fgv_sva_mode.vi"("cal_file_in"=w816, "mode"="Set (CAL-File)") -> ()  [unwired: 7 in, 3 out]
        }
        event Timeout {
          n425 = event-data() -> ()  [unwired: 1 in, 3 out]
        }
        event Panel Close? {
          w820 = "Plots" ("section")
          w901 = "Plots" ("section")
          w894 = "Plots" ("section")
          w871 = "Plots" ("section")
          w846 = "Plots" ("section")
          w912 = "Plots" ("section")
          w935 = "Plots" ("section")
          w956 = "Plots" ("section")
          w957 = "Siglent_SSA/SVA" ("section")
          # "Save User Settings"
          n426 = event-data() -> ()  [unwired: 1 in, 4 out]
          n427 = Send Notification(notification=TRUE ("element"), notifier=w977) -> ()  [unwired: 1 in, 2 out]
          n428 = local read "selector_serial_port"() -> (w975:refnum<visa-resource-name>)
          n429 = local read "color_picker_phase"() -> (w955:u32)
          n430 = local read "enable_plot_vswr"() -> (w853:bool)
          n431 = local read "color_picker_jx"() -> (w933:u32)
          n432 = local read "color_picker_cs"() -> (w914:u32)
          n433 = local read "enable_plot_rp"() -> (w873:bool)
          n434 = local read "enable_plot_lp"() -> (w892:bool)
          n435 = call <vilib>:"Application Directory.vi"() -> ("Application Directory"=w837:path)
          n436 = Build Path(base path=w837, name or relative path=path "data/plot_config.ini") -> (appended path=w841:path)
          n437 = call <vilib>:"Open Config Data.vi"("configuration file path"=w841) -> ("error out"=w839:errorcluster, "refnum"=w838:T7)  [unwired: 8 in, 1 out]
          n438 = call-poly <vilib>:"Write Key.vi"("section"="NanoVNA", "error in (no error)"=w839, "value"=w975, "key"="COM_Port", "refnum"=w838) -> ("error out"=w971:errorcluster, "refnum out"=w972:T7)  [unwired: 4 in, 1 out]
          n439 = local read "color_picker_vswr"() -> (w950:u32)
          n440 = local read "color_picker_rp"() -> (w930:u32)
          n441 = local read "color_picker_lp"() -> (w908:u32)
          n442 = local read "enable_plot_real"() -> (w856:bool)
          n443 = local read "enable_plot_jxp"() -> (w876:bool)
          n444 = local read "enable_plot_cp"() -> (w898:bool)
          n445 = local read "sva_ip"() -> (w970:string)
          n446 = call-poly <vilib>:"Write Key.vi"("section"=w957, "error in (no error)"=w971, "value"=w970, "key"="IP_Address", "refnum"=w972) -> ("error out"=w966:errorcluster, "refnum out"=w967:T7)  [unwired: 4 in, 1 out]
          n447 = property on="sva_cal_file" class="CmbBox"() -> ("Strings[]"=w831:string[])  [unwired: 2 in, 2 out]
          n448 = local read "enable_plot_imag"() -> (w859:bool)
          n449 = local read "color_picker_real"() -> (w947:u32)
          n450 = local read "color_picker_jxp"() -> (w925:u32)
          n451 = local read "color_picker_cp"() -> (w905:u32)
          n452 = local read "enable_plot_z"() -> (w881:bool)
          n453 = local read "sva_port"() -> (w969:u16)
          n454 = Array To Spreadsheet String(delimiter (Tab)=";", array=w831, 3:"%s" ("format string")) -> (spreadsheet string=w836:string)
          n455 = local read "color_picker_cursor_1"() -> (w827:u32)
          n456 = call-poly <vilib>:"Write Key.vi"("section"=w957, "error in (no error)"=w966, "value"=w969, "key"="Port", "refnum"=w967) -> ("error out"=w962:errorcluster, "refnum out"=w963:T7)  [unwired: 4 in, 1 out]
          n457 = local read "enable_plot_logmag"() -> (w847:bool)
          n458 = local read "color_picker_imag"() -> (w942:u32)
          n459 = local read "color_picker_z"() -> (w922:u32)
          n460 = local read "enable_plot_ls"() -> (w884:bool)
          n461 = local read "cursor_mode"() -> (w964:bool)
          n462 = local read "enable_plot_r"() -> (w864:bool)
          n463 = local read "color_picker_cursor_2"() -> (w826:u32)
          n464 = call-poly <vilib>:"Write Key.vi"("section"=w956, "error in (no error)"=w962, "value"=w964, "key"="Cursor_Interlock", "refnum"=w963) -> ("error out"=w958:errorcluster, "refnum out"=w959:T7)  [unwired: 4 in, 1 out]
          n465 = local read "color_picker_logmag"() -> (w961:u32)
          n466 = local read "enable_plot_phase"() -> (w850:bool)
          n467 = local read "color_picker_ls"() -> (w917:u32)
          n468 = local read "enable_plot_jx"() -> (w867:bool)
          n469 = local read "enable_plot_cs"() -> (w889:bool)
          n470 = local read "color_picker_r"() -> (w939:u32)
          n471 = call-poly <vilib>:"Write Key.vi"("section"=w956, "error in (no error)"=w958, "value"=w961, "key"="Color_Plot_0_0", "refnum"=w959) -> ("error out"=w952:errorcluster, "refnum out"=w953:T7)  [unwired: 4 in, 1 out]
          n472 = call-poly <vilib>:"Write Key.vi"("section"=w935, "error in (no error)"=w952, "value"=w955, "key"="Color_Plot_0_1", "refnum"=w953) -> ("error out"=w948:errorcluster, "refnum out"=w949:T7)  [unwired: 4 in, 1 out]
          n473 = call-poly <vilib>:"Write Key.vi"("section"=w935, "error in (no error)"=w948, "value"=w950, "key"="Color_Plot_0_2", "refnum"=w949) -> ("error out"=w944:errorcluster, "refnum out"=w945:T7)  [unwired: 4 in, 1 out]
          n474 = call-poly <vilib>:"Write Key.vi"("section"=w935, "error in (no error)"=w944, "value"=w947, "key"="Color_Plot_1_0", "refnum"=w945) -> ("error out"=w940:errorcluster, "refnum out"=w941:T7)  [unwired: 4 in, 1 out]
          n475 = call-poly <vilib>:"Write Key.vi"("section"=w935, "error in (no error)"=w940, "value"=w942, "key"="Color_Plot_1_1", "refnum"=w941) -> ("error out"=w936:errorcluster, "refnum out"=w937:T7)  [unwired: 4 in, 1 out]
          n476 = call-poly <vilib>:"Write Key.vi"("section"=w935, "error in (no error)"=w936, "value"=w939, "key"="Color_Plot_2_0", "refnum"=w937) -> ("error out"=w931:errorcluster, "refnum out"=w932:T7)  [unwired: 4 in, 1 out]
          n477 = call-poly <vilib>:"Write Key.vi"("section"=w912, "error in (no error)"=w931, "value"=w933, "key"="Color_Plot_2_1", "refnum"=w932) -> ("error out"=w927:errorcluster, "refnum out"=w928:T7)  [unwired: 4 in, 1 out]
          n478 = call-poly <vilib>:"Write Key.vi"("section"=w912, "error in (no error)"=w927, "value"=w930, "key"="Color_Plot_2_2", "refnum"=w928) -> ("error out"=w923:errorcluster, "refnum out"=w924:T7)  [unwired: 4 in, 1 out]
          n479 = call-poly <vilib>:"Write Key.vi"("section"=w912, "error in (no error)"=w923, "value"=w925, "key"="Color_Plot_2_3", "refnum"=w924) -> ("error out"=w919:errorcluster, "refnum out"=w920:T7)  [unwired: 4 in, 1 out]
          n480 = call-poly <vilib>:"Write Key.vi"("section"=w912, "error in (no error)"=w919, "value"=w922, "key"="Color_Plot_2_4", "refnum"=w920) -> ("error out"=w915:errorcluster, "refnum out"=w916:T7)  [unwired: 4 in, 1 out]
          n481 = call-poly <vilib>:"Write Key.vi"("section"=w912, "error in (no error)"=w915, "value"=w917, "key"="Color_Plot_3_0", "refnum"=w916) -> ("error out"=w910:errorcluster, "refnum out"=w911:T7)  [unwired: 4 in, 1 out]
          n482 = call-poly <vilib>:"Write Key.vi"("section"=w846, "error in (no error)"=w910, "value"=w914, "key"="Color_Plot_3_1", "refnum"=w911) -> ("error out"=w906:errorcluster, "refnum out"=w907:T7)  [unwired: 4 in, 1 out]
          n483 = call-poly <vilib>:"Write Key.vi"("section"=w846, "error in (no error)"=w906, "value"=w908, "key"="Color_Plot_3_2", "refnum"=w907) -> ("error out"=w902:errorcluster, "refnum out"=w903:T7)  [unwired: 4 in, 1 out]
          n484 = call-poly <vilib>:"Write Key.vi"("section"=w846, "error in (no error)"=w902, "value"=w905, "key"="Color_Plot_3_3", "refnum"=w903) -> ("error out"=w842:errorcluster, "refnum out"=w843:T7)  [unwired: 4 in, 1 out]
          n485 = call-poly <vilib>:"Write Key.vi"("section"=w846, "error in (no error)"=w842, "value"=w847, "key"="Enable_Plot_0_0", "refnum"=w843) -> ("error out"=w852:errorcluster, "refnum out"=w851:T7)  [unwired: 4 in, 1 out]
          n486 = call-poly <vilib>:"Write Key.vi"("section"=w846, "error in (no error)"=w852, "value"=w850, "key"="Enable_Plot_0_1", "refnum"=w851) -> ("error out"=w845:errorcluster, "refnum out"=w844:T7)  [unwired: 4 in, 1 out]
          n487 = call-poly <vilib>:"Write Key.vi"("section"=w871, "error in (no error)"=w845, "value"=w853, "key"="Enable_Plot_0_2", "refnum"=w844) -> ("error out"=w858:errorcluster, "refnum out"=w857:T7)  [unwired: 4 in, 1 out]
          n488 = call-poly <vilib>:"Write Key.vi"("section"=w871, "error in (no error)"=w858, "value"=w856, "key"="Enable_Plot_1_0", "refnum"=w857) -> ("error out"=w862:errorcluster, "refnum out"=w861:T7)  [unwired: 4 in, 1 out]
          n489 = call-poly <vilib>:"Write Key.vi"("section"=w871, "error in (no error)"=w862, "value"=w859, "key"="Enable_Plot_1_1", "refnum"=w861) -> ("error out"=w866:errorcluster, "refnum out"=w865:T7)  [unwired: 4 in, 1 out]
          n490 = call-poly <vilib>:"Write Key.vi"("section"=w871, "error in (no error)"=w866, "value"=w864, "key"="Enable_Plot_2_0", "refnum"=w865) -> ("error out"=w870:errorcluster, "refnum out"=w869:T7)  [unwired: 4 in, 1 out]
          n491 = call-poly <vilib>:"Write Key.vi"("section"=w871, "error in (no error)"=w870, "value"=w867, "key"="Enable_Plot_2_1", "refnum"=w869) -> ("error out"=w875:errorcluster, "refnum out"=w874:T7)  [unwired: 4 in, 1 out]
          n492 = call-poly <vilib>:"Write Key.vi"("section"=w894, "error in (no error)"=w875, "value"=w873, "key"="Enable_Plot_2_2", "refnum"=w874) -> ("error out"=w879:errorcluster, "refnum out"=w878:T7)  [unwired: 4 in, 1 out]
          n493 = call-poly <vilib>:"Write Key.vi"("section"=w894, "error in (no error)"=w879, "value"=w876, "key"="Enable_Plot_2_3", "refnum"=w878) -> ("error out"=w883:errorcluster, "refnum out"=w882:T7)  [unwired: 4 in, 1 out]
          n494 = call-poly <vilib>:"Write Key.vi"("section"=w894, "error in (no error)"=w883, "value"=w881, "key"="Enable_Plot_2_4", "refnum"=w882) -> ("error out"=w887:errorcluster, "refnum out"=w886:T7)  [unwired: 4 in, 1 out]
          n495 = call-poly <vilib>:"Write Key.vi"("section"=w894, "error in (no error)"=w887, "value"=w884, "key"="Enable_Plot_3_0", "refnum"=w886) -> ("error out"=w891:errorcluster, "refnum out"=w890:T7)  [unwired: 4 in, 1 out]
          n496 = call-poly <vilib>:"Write Key.vi"("section"=w894, "error in (no error)"=w891, "value"=w889, "key"="Enable_Plot_3_1", "refnum"=w890) -> ("error out"=w896:errorcluster, "refnum out"=w895:T7)  [unwired: 4 in, 1 out]
          n497 = call-poly <vilib>:"Write Key.vi"("section"=w901, "error in (no error)"=w896, "value"=w892, "key"="Enable_Plot_3_2", "refnum"=w895) -> ("error out"=w900:errorcluster, "refnum out"=w899:T7)  [unwired: 4 in, 1 out]
          n498 = call-poly <vilib>:"Write Key.vi"("section"=w901, "error in (no error)"=w900, "value"=w898, "key"="Enable_Plot_3_3", "refnum"=w899) -> ("error out"=w834:errorcluster, "refnum out"=w835:T7)  [unwired: 4 in, 1 out]
          n499 = call-poly <vilib>:"Write Key.vi"("section"="Siglent_SSA/SVA", "error in (no error)"=w834, "value"=w836, "key"="CAL-File_History", "refnum"=w835) -> ("error out"=w823:errorcluster, "refnum out"=w824:T7)  [unwired: 4 in, 1 out]
          n500 = call-poly <vilib>:"Write Key.vi"("section"=w820, "error in (no error)"=w823, "value"=w827, "key"="Color_Cursor_1", "refnum"=w824) -> ("error out"=w822:errorcluster, "refnum out"=w821:T7)  [unwired: 4 in, 1 out]
          n501 = call-poly <vilib>:"Write Key.vi"("section"=w820, "error in (no error)"=w822, "value"=w826, "key"="Color_Cursor_2", "refnum"=w821) -> ("error out"=w818:errorcluster, "refnum out"=w819:T7)  [unwired: 4 in, 1 out]
          n502 = call <vilib>:"Close Config Data.vi"("error in (no error)"=w818, "refnum"=w819) -> ()  [unwired: 8 in, 2 out]
          n503 = event-data() -> ()  [unwired: 2 in, 1 out]
        }
      }
      n504 = case shown="True" w424 {
        frame False {
        }
        frame True {
          n505 = call "fgv_cursor_data.vi"() -> ("cursor_idx_get"=w446:i32, "cursor_data_get"=w443:T13)  [unwired: 9 in, 5 out]
          n506 = Unbundle(w443) -> ("cursor_data"=w450:dbl[], "frequency"=w445:string, "wavelength_m"=w444:dbl)
          n507 = Index Array(array=w450) -> (element #1=w447:dbl, element #2=w448:dbl, element #3=w449:dbl)  [unwired: 3 in]
          n508 = case shown="0, Default" w446 {
            tunnel: w449 -> [w453 w460]
            tunnel: w448 -> [w452 w459]
            tunnel: w447 -> [w451 w458]
            tunnel: w445 -> [w454 w457]
            tunnel: w444 -> [w455 w456]
            frame 0, Default {
              n509 = local write "cursor_logmag_1"(w451) -> ()
              n510 = local write "cursor_phase_1"(w452) -> ()
              n511 = local write "cursor_vswr_1"(w453) -> ()
              n512 = local write "cursor_log_phase_freq_1"(w454) -> ()
              n513 = local write "cursor_log_phase_wavel_1"(w455) -> ()
            }
            frame 1 {
              n514 = local write "cursor_logmag_2"(w458) -> ()
              n515 = local write "cursor_phase_2"(w459) -> ()
              n516 = local write "cursor_vswr_2"(w460) -> ()
              n517 = local write "cursor_log_phase_freq_2"(w457) -> ()
              n518 = local write "cursor_log_phase_wavel_2"(w456) -> ()
            }
          }
        }
      }
      n519 = case shown="True" w423 {
        frame False {
        }
        frame True {
          n520 = call "fgv_cursor_data.vi"() -> ("cursor_idx_get"=w433:i32, "cursor_data_get"=w428:T13)  [unwired: 9 in, 5 out]
          n521 = Unbundle(w428) -> ("cursor_data"=w434:dbl[], "frequency"=w430:string, "wavelength_m"=w429:dbl)
          n522 = Index Array(array=w434) -> (element #1=w432:dbl, element #2=w431:dbl)  [unwired: 2 in]
          n523 = case shown="0, Default" w433 {
            tunnel: w432 -> [w438 w442]
            tunnel: w431 -> [w437 w441]
            tunnel: w430 -> [w436 w440]
            tunnel: w429 -> [w435 w439]
            frame 0, Default {
              n524 = local write "cursor_real_1"(w438) -> ()
              n525 = local write "cursor_imag_1"(w437) -> ()
              n526 = local write "cursor_real_imag_freq_1"(w436) -> ()
              n527 = local write "cursor_real_imag_wavel_1"(w435) -> ()
            }
            frame 1 {
              n528 = local write "cursor_real_2"(w442) -> ()
              n529 = local write "cursor_imag_2"(w441) -> ()
              n530 = local write "cursor_real_imag_freq_2"(w440) -> ()
              n531 = local write "cursor_real_imag_wavel_2"(w439) -> ()
            }
          }
        }
      }
    }
    n532 = call "Is Value Changed.vim"("value"=w62) -> ("changed or first call?"=w60:bool)
    n533 = call "Is Value Changed.vim"("value"=w47) -> ("changed or first call?"=w58:bool)
    n534 = And(x=w58, y=w47) -> (x .and. y?=w59:bool)
    n535 = Or(x=w60, y=w59) -> (x .or. y?=w61:bool)
    n536 = Or(x=w47, y=w48) -> (x .or. y?=w49:bool)
    n537 = case shown="True" w49 {
      frame False {
        n538 = property on="button_single_sweep" class="Bool"("DisabledEnum"=T3."Disabled and Grayed Out" ("Disabled")) -> ()  [unwired: 2 in, 2 out]
        n539 = property on="button_auto_sweep" class="Bool (strict)"("DisabledEnum"=T3."Disabled and Grayed Out" ("Disabled")) -> ()  [unwired: 2 in, 2 out]
      }
      frame True {
        n540 = property on="button_auto_sweep" class="Bool (strict)"("DisabledEnum"=T3."Enabled" ("Disabled")) -> ("Value"=w178:bool)  [unwired: 2 in, 2 out]
        n541 = case shown="False" w178 {
          tunnel: [T3."Enabled" ("Disabled") T3."Disabled and Grayed Out" ("Disabled")] -> w179
          frame False {
          }
          frame True {
          }
        }
        n542 = property on="button_single_sweep" class="Bool"("DisabledEnum"=w179) -> ()  [unwired: 2 in, 2 out]
      }
    }
    n543 = case shown="True" w48 {
      frame False {
        w411 = T3."Enabled" ("Disabled")
        n544 = property on="selector_serial_port" class="VISAName"("DisabledEnum"=w411) -> ()  [unwired: 2 in, 2 out]
        n545 = property on="button_tcp_connect" class="Bool (strict)"("DisabledEnum"=w411) -> ()  [unwired: 2 in, 2 out]
      }
      frame True {
        w412 = T3."Disabled and Grayed Out" ("Disabled")
        n546 = property on="selector_serial_port" class="VISAName"("DisabledEnum"=w412) -> ()  [unwired: 2 in, 2 out]
        n547 = property on="button_tcp_connect" class="Bool (strict)"("DisabledEnum"=w412) -> ()  [unwired: 2 in, 2 out]
      }
    }
    n548 = case shown="True" w61 {
      tunnel: w62 -> [_ w209]
      frame False {
      }
      frame True {
        n549 = Unbundle(w209) -> ("mode"=w208:string, "s11_s21"=w207:string, "graph"=w206:string, "freq_range"=w200:cluster{"start_freq":string, "stop_freq":string}, "points"=w199:string)
        n550 = case shown="\"VNA\"" w208 {
          tunnel: [T3."Disabled and Grayed Out" ("DisabledEnum") T3."Enabled" ("DisabledEnum")] -> w201
          tunnel: [cluster{u32, u32}[] [{16711680, 16711680}, {4424887, 4424887}, {4424887, 4424887}, {4424887, 4424887}, {4424887, 16777215}, {4424887, 16777215}] ("Colors [4]") cluster{u32, u32}[] [{6618880, 6618880}, {4424887, 4424887}, {4424887, 4424887}, {4424887, 4424887}, {4424887, 16777215}, {4424887, 16777215}] ("Colors [4]")] -> w205
          tunnel: w200 -> [_ w223]
          tunnel: w199 -> [_ w222]
          frame "SA", Default {
          }
          frame "VNA" {
            n551 = call "tcp_sweep_preset.vi"("points_in"=w222, "freq_range"=w223) -> ("points_out"=w219:i32, "stop_freq"=w220:dbl, "start_freq"=w221:dbl)  [unwired: 7 in]
            n552 = local write "sweep_start"(w221) -> ()
            n553 = local write "sweep_stop"(w220) -> ()
            n554 = local write "sweep_points"(w219) -> ()
          }
        }
        n555 = case shown="\"S21\"" w207 {
          tunnel: [w212 cluster{u32, u32}[] [{6618880, 6618880}, {4424887, 4424887}, {4424887, 4424887}, {4424887, 4424887}, {4424887, 16777215}, {4424887, 16777215}] ("Colors [4]") cluster{u32, u32}[] [{11053998, 11053998}, {4424887, 4424887}, {4424887, 4424887}, {4424887, 4424887}, {4424887, 16777215}, {4424887, 16777215}] ("Colors [4]")] -> w204
          tunnel: [w212 cluster{u32, u32}[] [{11053998, 11053998}, {4424887, 4424887}, {4424887, 4424887}, {4424887, 4424887}, {4424887, 16777215}, {4424887, 16777215}] ("Colors [4]") cluster{u32, u32}[] [{6618880, 6618880}, {4424887, 4424887}, {4424887, 4424887}, {4424887, 4424887}, {4424887, 16777215}, {4424887, 16777215}] ("Colors [4]")] -> w203
          frame Default {
            w212 = cluster{u32, u32}[] [{11053998, 11053998}, {4424887, 4424887}, {4424887, 4424887}, {4424887, 4424887}, {4424887, 16777215}, {4424887, 16777215}] ("Colors [4]")
          }
          frame "S11" {
          }
          frame "S21" {
          }
        }
        n556 = case shown="\"SMIT\"" w206 {
          tunnel: [cluster{u32, u32}[] [{16711680, 16711680}, {4424887, 4424887}, {4424887, 4424887}, {4424887, 4424887}, {4424887, 16777215}, {4424887, 16777215}] ("Colors [4]") cluster{u32, u32}[] [{6618880, 6618880}, {4424887, 4424887}, {4424887, 4424887}, {4424887, 4424887}, {4424887, 16777215}, {4424887, 16777215}] ("Colors [4]")] -> w202
          frame "MLOG", Default {
          }
          frame "SMIT" {
          }
        }
        n557 = property on="button_tcp_vna_mode" class="Bool"("Colors [4]"=w205) -> ()  [unwired: 2 in, 2 out]
        n558 = property on="button_tcp_load_cal" class="Bool"("DisabledEnum"=w201) -> ()  [unwired: 2 in, 2 out]
        n559 = property on="button_tcp_s11_mode" class="Bool"("Colors [4]"=w204, "DisabledEnum"=w201) -> ()  [unwired: 2 in, 2 out]
        n560 = property on="button_tcp_s21_mode" class="Bool"("Colors [4]"=w203, "DisabledEnum"=w201) -> ()  [unwired: 2 in, 2 out]
        n561 = property on="button_tcp_smith_mode" class="Bool"("Colors [4]"=w202, "DisabledEnum"=w201) -> ()  [unwired: 2 in, 2 out]
      }
    }
    n562 = case shown="True" "show_smith_window" {
      selector: "show_smith_window" -> [w416 w417]
      tunnel: "show_smith_window" -> [_ w419]
      tunnel: [w416 w418] -> w74
      frame False {
        (unwired) FALSE ("show_smith_window")
      }
      frame True {
        n563 = Open VI Reference(vi path=path "02_ui_smith_plot.vi") -> (vi reference=w421:refnum<vi>)  [unwired: 5 in, 1 out]
        n564 = invoke class="VI" method="FP.Open"(reference=w421, "Activate"=w419, "State"=T4."Standard") -> ()  [unwired: 2 in, 5 out]
        n565 = Not(x=w417) -> (.not. x?=w418:bool)
      }
    }
    n566 = case shown="True" "show_plot_window" {
      tunnel: "show_plot_window" -> [_ w391]
      frame False {
      }
      frame True {
        n567 = Open VI Reference(vi path=path "02_ui_plot_window.vi") -> (vi reference=w393:refnum<vi>)  [unwired: 5 in, 1 out]
        n568 = invoke class="VI" method="FP.Open"(reference=w393, "Activate"=w391, "State"=T4."Standard") -> ()  [unwired: 2 in, 5 out]
      }
    }
    n569 = call "Is Value Changed.vim"("value"="sva_port") -> ("changed or first call?"=w84:bool)
    n570 = call "Is Value Changed.vim"("value"="sva_ip") -> ("changed or first call?"=w83:bool)
    n571 = Or(x=w84, y=w83) -> (x .or. y?=w85:bool)
    n572 = case shown="True" w85 {
      tunnel: "sva_ip" -> [_ w390]
      tunnel: "sva_port" -> [_ w389]
      frame False {
      }
      frame True {
        n573 = call "fgv_tcp_con_param.vi"("mode"="Set (IP/Port)", "port_set"=w389, "ip_address_set"=w390) -> ()  [unwired: 5 in, 4 out]
      }
    }
    n574 = local write "show_smith_window"(w74) -> ()
    n575 = control-ref of="plot_log_phase_vswr"() -> (w110:refnum<vi>)
    n576 = control-ref of="plot_real_imag"() -> (w104:refnum<vi>)
    n577 = call "show_plot.vi"("plot_id"=0 ("y_scale_id"), "show_plot"="enable_plot_logmag", "XYGraph Refnum"=w110) -> ()  [unwired: 8 in, 1 out]
    n578 = call "show_plot.vi"("plot_id"=1 ("y_scale_id"), "show_plot"="enable_plot_phase", "XYGraph Refnum"=w110) -> ()  [unwired: 8 in, 1 out]
    n579 = call "show_plot.vi"("plot_id"=2 ("y_scale_id"), "show_plot"="enable_plot_vswr", "XYGraph Refnum"=w110) -> ()  [unwired: 8 in, 1 out]
    n580 = local read "set_min_vswr_c2"() -> (w23:bool)
    n581 = local read "set_min_vswr_c1"() -> (w26:bool)
    n582 = case shown="True" w26 {
      tunnel: [_ w173] -> w38
      tunnel: [_ 0 ("CursIdx")] -> w37
      tunnel: [w168 99 ("plot_id_get")] -> w35
      tunnel: [_ "Set (Cursor Data)"] -> w24
      frame False {
        n583 = call "fgv_cursor_data.vi"() -> ("plot_id_get"=w168:i32)  [unwired: 9 in, 6 out]
      }
      frame True {
        n584 = local write "set_min_vswr_c1"(FALSE ("set_c1")) -> ()
        n585 = local read "min_vswr_idx"() -> (w173:i32)
      }
    }
    n586 = case shown="True" w23 {
      tunnel: [w161 w165] -> w28
      tunnel: [w162 1 ("CursIdx")] -> w27
      tunnel: w37 -> [w162 _]
      tunnel: w38 -> [w161 _]
      tunnel: [w160 99 ("plot_id_get")] -> w36
      tunnel: w35 -> [w160 _]
      tunnel: w24 -> [w159 _]
      tunnel: [w159 "Set (Cursor Data)"] -> w22
      frame False {
      }
      frame True {
        n587 = local write "set_min_vswr_c2"(FALSE ("set_c1")) -> ()
        n588 = local read "min_vswr_idx"() -> (w165:i32)
      }
    }
    n589 = call "show_plot.vi"("plot_id"=0 ("y_scale_id"), "autoscale"=FALSE, "show_plot"="enable_plot_real", "XYGraph Refnum"=w104) -> ()  [unwired: 7 in, 1 out]
    n590 = call "show_plot.vi"("plot_id"=1 ("y_scale_id"), "autoscale"=FALSE, "show_plot"="enable_plot_imag", "XYGraph Refnum"=w104) -> ()  [unwired: 7 in, 1 out]
    n591 = call "Is Value Changed.vim"("value"="cursor_mode") -> ("changed or first call?"=w32:bool)
    n592 = case shown="True" w32 {
      tunnel: "cursor_mode" -> [_ w135]
      frame False {
      }
      frame True {
        n593 = call "fgv_cursor_data.vi"("cursor_mode_set"=w135, "mode"="Set (Cursor Mode)") -> ()  [unwired: 7 in, 7 out]
      }
    }
    n594 = call "fgv_freq_real_imag.vi"() -> ("plot_data"=w78:T14, "data_array_get"=w79:dbl[][], "freq_array_get"=w77:dbl[])  [unwired: 8 in, 1 out]
    n595 = call "Is Value Changed.vim"("value"=w79) -> ("changed or first call?"=w76:bool)
    n596 = control-ref of="plot_rjx"() -> (w124:refnum<vi>)
    n597 = case shown="True" w76 {
      tunnel: [FALSE TRUE] -> w116
      tunnel: w78 -> [_ w985]
      tunnel: w77 -> [_ w984]
      frame False {
      }
      frame True {
        w1009 = i16 0 ("Precision")
        # "R+jX_Norm"
        # "L/C"
        # "R/jX"
        # "Real/Imag"
        # "Log/Phase/VSWR"
        n598 = Array Subset(array=w985, index=17, length=2) -> (w980:T14)
        n599 = Array Subset(array=w985, index=0, length=3) -> (w996:T14)
        n600 = Array Subset(array=w985, index=3, length=2) -> (w981:T14)
        n601 = Array Subset(array=w985, index=5, length=5) -> (w991:T14)
        n602 = Array Subset(array=w985, index=10, length=4) -> (w988:T14)
        n603 = call "calc_plot_to_smith.vi"("Plot_Data"=w980) -> ("smith plot"=w983:cluster{"r":dbl, "x":dbl}[])  [unwired: 10 in]
        n604 = Array Size(array=w984) -> (size(s)=w1010:i32)
        n605 = Array Max & Min(array=w984) -> (max value=w1007:dbl, min value=w1008:dbl)  [unwired: 2 out]
        n606 = call "prepare_smith_plot.vi"("dimensions (w,h)"=cluster{"width":i16, "height":i16} {"width"=600, "height"=600}, "smith plot"=w983) -> ("smith_out"=w999:picture)  [unwired: 9 in]
        n607 = local write "points"(w1010) -> ()
        n608 = property on="plot_smith" class="Pict"("Val(Sgnl)"=w999) -> ()  [unwired: 2 in, 2 out]
        n609 = property on="plot_log_phase_vswr" class="XYGraph (strict)"("Val(Sgnl)"=w996) -> ()  [unwired: 2 in, 2 out]
        n610 = property on="plot_rjx" class="XYGraph (strict)"("Val(Sgnl)"=w991) -> ()  [unwired: 2 in, 2 out]
        n611 = property on="plot_real_imag" class="XYGraph (strict)"("Val(Sgnl)"=w981) -> ()  [unwired: 2 in, 2 out]
        n612 = property on="plot_lc" class="XYGraph (strict)"("Val(Sgnl)"=w988) -> ()  [unwired: 2 in, 2 out]
        n613 = call "number_with_decimal_points.vi"("Precision"=w1009, "Double"=w1007) -> ("String"=w1005:string)  [unwired: 5 in]
        n614 = call "calc_min_vswr.vi"("plot_log_phase_vswr"=w996) -> ("min_vswr_idx"=→"min_vswr_idx":i32, "min_vswr"=w1001:dbl, "min_vswr_freq"=w1004:string)  [unwired: 8 in]
        n615 = call "number_with_decimal_points.vi"("Precision"=w1009, "Double"=w1008) -> ("String"=w1006:string)  [unwired: 5 in]
        n616 = local write "max_frequency"(w1005) -> ()
        n617 = local write "min_frequency"(w1006) -> ()
        n618 = local write "min_vswr_freq"(w1004) -> ()
        n619 = local write "min_vswr"(w1001) -> ()
        n620 = disable-structure shown="Disabled" {
          frame Disabled {
            # "Anpass Linien einzeichnen"
            # "Smith Scale"
            n621 = call <vilib>:"Draw Standard Smith Grid.vi"("Clip Rect"=T5 {"left"=600.0, "top"=0.0, "right"=0.0, "bottom"=600.0}, 9:FALSE ("Show minor"), "Scale Factors"=T6 {"x"={"a"=300.0, "b"=300.0, "log?"=FALSE}, "y"={"a"=-300.0, "b"=300.0, "log?"=FALSE}}) -> ()  [unwired: 8 in, 1 out]
            n622 = call <vilib>:"Draw Smith PolyLine.vi"() -> ()  [unwired: 11 in, 1 out]
          }
          frame Enabled {
          }
        }
        n623 = call "fgv_load_save.vi"() -> ("filename_get"=→"filename":string)  [unwired: 10 in, 1 out]
      }
    }
    n624 = call "set_plot_rjx.vi"("enable_plot_jx"="enable_plot_jx", "set_scale"=w116, "enable_plot_jxp"="enable_plot_jxp", "enable_plot_r"="enable_plot_r", "enable_plot_rp"="enable_plot_rp", "enable_plot_z"="enable_plot_z", "plot_rjx_ref"=w124, "rx_scale_settings"="rx_scale_settings") -> ()  [unwired: 8 in]
    n625 = call "fgv_cursor_data.vi"("cursor_idx_set"=w27, "cursor_pos_set"=w28, "mode"=w22) -> ("cursor_idx_get"=w30:i32, "cursor_pos_get"=w29:i32, "cursor_mode_get"=w33:bool)  [unwired: 6 in, 4 out]
    n626 = call "Is Value Changed.vim"("value"=w29) -> ("changed or first call?"=w25:bool)
    n627 = control-ref of="plot_lc"() -> (w118:refnum<vi>)
    n628 = And(x=w25, y=w33) -> (x .and. y?=w34:bool)
    n629 = call "set_plot_lc.vi"("lc_scale_settings"="lc_scale_settings", "plot_lc_ref"=w118, "set_scale"=w116, "enable_plot_lp"="enable_plot_lp", "enable_plot_ls"="enable_plot_ls", "enable_plot_cp"="enable_plot_cp", "enable_plot_cs"="enable_plot_cs") -> ()  [unwired: 5 in]
    n630 = case shown="True" w34 {
      tunnel: w30 -> [_ w138]
      tunnel: w29 -> [_ w139]
      tunnel: w36 -> [_ w137]
      frame False {
      }
      frame True {
        n631 = local read "plot_rjx"() -> (w140:cluster{"array type (2D Dbl)":dbl[], dbl[]}[])
        n632 = control-ref of="plot_smith"() -> (w141:refnum<vi>)
        n633 = case shown="99, Default" w137 {
          tunnel: w138 -> [_ w158]
          tunnel: w139 -> [_ w157]
          frame 0 {
          }
          frame 99, Default {
            n634 = property on="plot_log_phase_vswr" class="XYGraph (strict)"("Active Cursor"=w158, "Cursor.Cursor Index"=w157) -> (error out=w155:errorcluster, "Value"=w156:cluster{"array type (2D Dbl)":dbl[], dbl[]}[])  [unwired: 2 in, 1 out]
            n635 = property on="plot_log_phase_vswr" class="XYGraph (strict)"(error in=w155, "Val(Sgnl)"=w156) -> ()  [unwired: 1 in, 2 out]
          }
        }
        n636 = case shown="99, Default" w137 {
          tunnel: w138 -> [w154 _]
          tunnel: w139 -> [w153 _]
          frame 99, Default {
            n637 = property on="plot_real_imag" class="XYGraph (strict)"("Active Cursor"=w154, "Cursor.Cursor Index"=w153) -> (error out=w151:errorcluster, "Value"=w152:cluster{"array type (2D Dbl)":dbl[], dbl[]}[])  [unwired: 2 in, 1 out]
            n638 = property on="plot_real_imag" class="XYGraph (strict)"(error in=w151, "Val(Sgnl)"=w152) -> ()  [unwired: 1 in, 2 out]
          }
          frame 1 {
          }
        }
        n639 = case shown="99, Default" w137 {
          tunnel: w138 -> [w150 _]
          tunnel: w139 -> [w149 _]
          frame 99, Default {
            n640 = property on="plot_rjx" class="XYGraph (strict)"("Active Cursor"=w150, "Cursor.Cursor Index"=w149) -> (error out=w147:errorcluster, "Value"=w148:cluster{"array type (2D Dbl)":dbl[], dbl[]}[])  [unwired: 2 in, 1 out]
            n641 = property on="plot_rjx" class="XYGraph (strict)"(error in=w147, "Val(Sgnl)"=w148) -> ()  [unwired: 1 in, 2 out]
          }
          frame 2 {
          }
        }
        n642 = case shown="99, Default" w137 {
          tunnel: w138 -> [w146 _]
          tunnel: w139 -> [w145 _]
          frame 99, Default {
            n643 = property on="plot_lc" class="XYGraph (strict)"("Active Cursor"=w146, "Cursor.Cursor Index"=w145) -> (error out=w143:errorcluster, "Value"=w144:cluster{"array type (2D Dbl)":dbl[], dbl[]}[])  [unwired: 2 in, 1 out]
            n644 = property on="plot_lc" class="XYGraph (strict)"(error in=w143, "Val(Sgnl)"=w144) -> ()  [unwired: 1 in, 2 out]
          }
          frame 3 {
          }
        }
        n645 = Current VI's Path() -> (path=w142:path)
        n646 = call "set_smith_cursor_plot.vi"("path"=w142, "smith_plot"=w141, "cursor_pos"=w139, "cursor_index"=w138, "plot_rjx"=w140) -> ()  [unwired: 7 in]
      }
    }
    n647 = Wait (ms)(milliseconds to wait=u32 15) -> ()  [unwired: 1 out]
  }
  n648 = Release Notifier(notifier=w18) -> ()  [unwired: 2 in, 3 out]
  n649 = Release Notifier(notifier=w9) -> ()  [unwired: 2 in, 3 out]
  n650 = Release Notifier(notifier=w10) -> ()  [unwired: 2 in, 3 out]
  n651 = Release Notifier(notifier=w4) -> ()  [unwired: 2 in, 3 out]
  n652 = Release Notifier(notifier=w17) -> ()  [unwired: 2 in, 3 out]
  n653 = call "02_get_load_save.vi"() -> ()  [unwired: 12 in]
  n654 = call "02_ui_smith_plot.vi"() -> ()  [unwired: 12 in]
  n655 = call "02_ui_plot_window.vi"() -> ()  [unwired: 12 in]
